vi "GDSProject_CreateClass.vi"(0 "Project Refnum In":refnum<vi>, 1 "Project Item To Create Class Below(Use MyComputer if not wired)":refnum<vi>, 2 "ClassFolder":path=path "C:/Documents and Settings/Micke/Mina dokument/LabView/8.1 Beta/Projects/ClassFiles/MyClass3.lvclass", 3 "ClassName":string, 5 "error in (no error)":errorcluster) -> (14 "Project Refnum Out":refnum<vi>, 15 "Class Refnum Out":refnum<vi>, 16 "ClassPathOut":path, 19 "error out":errorcluster)   [LabVIEW 2020]
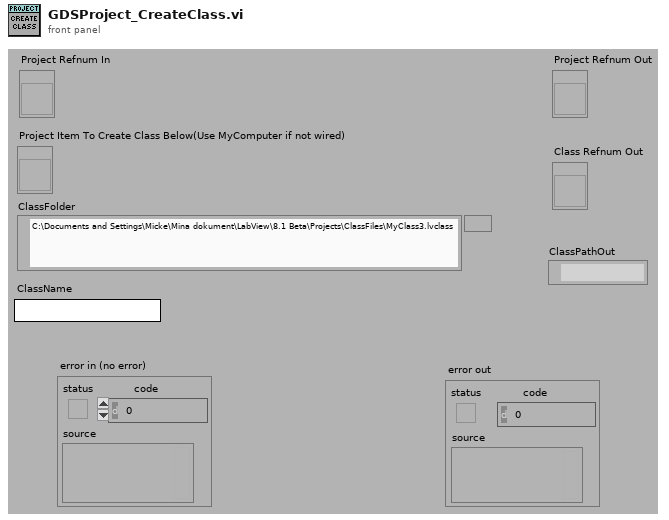
[diagram p1: front panel]
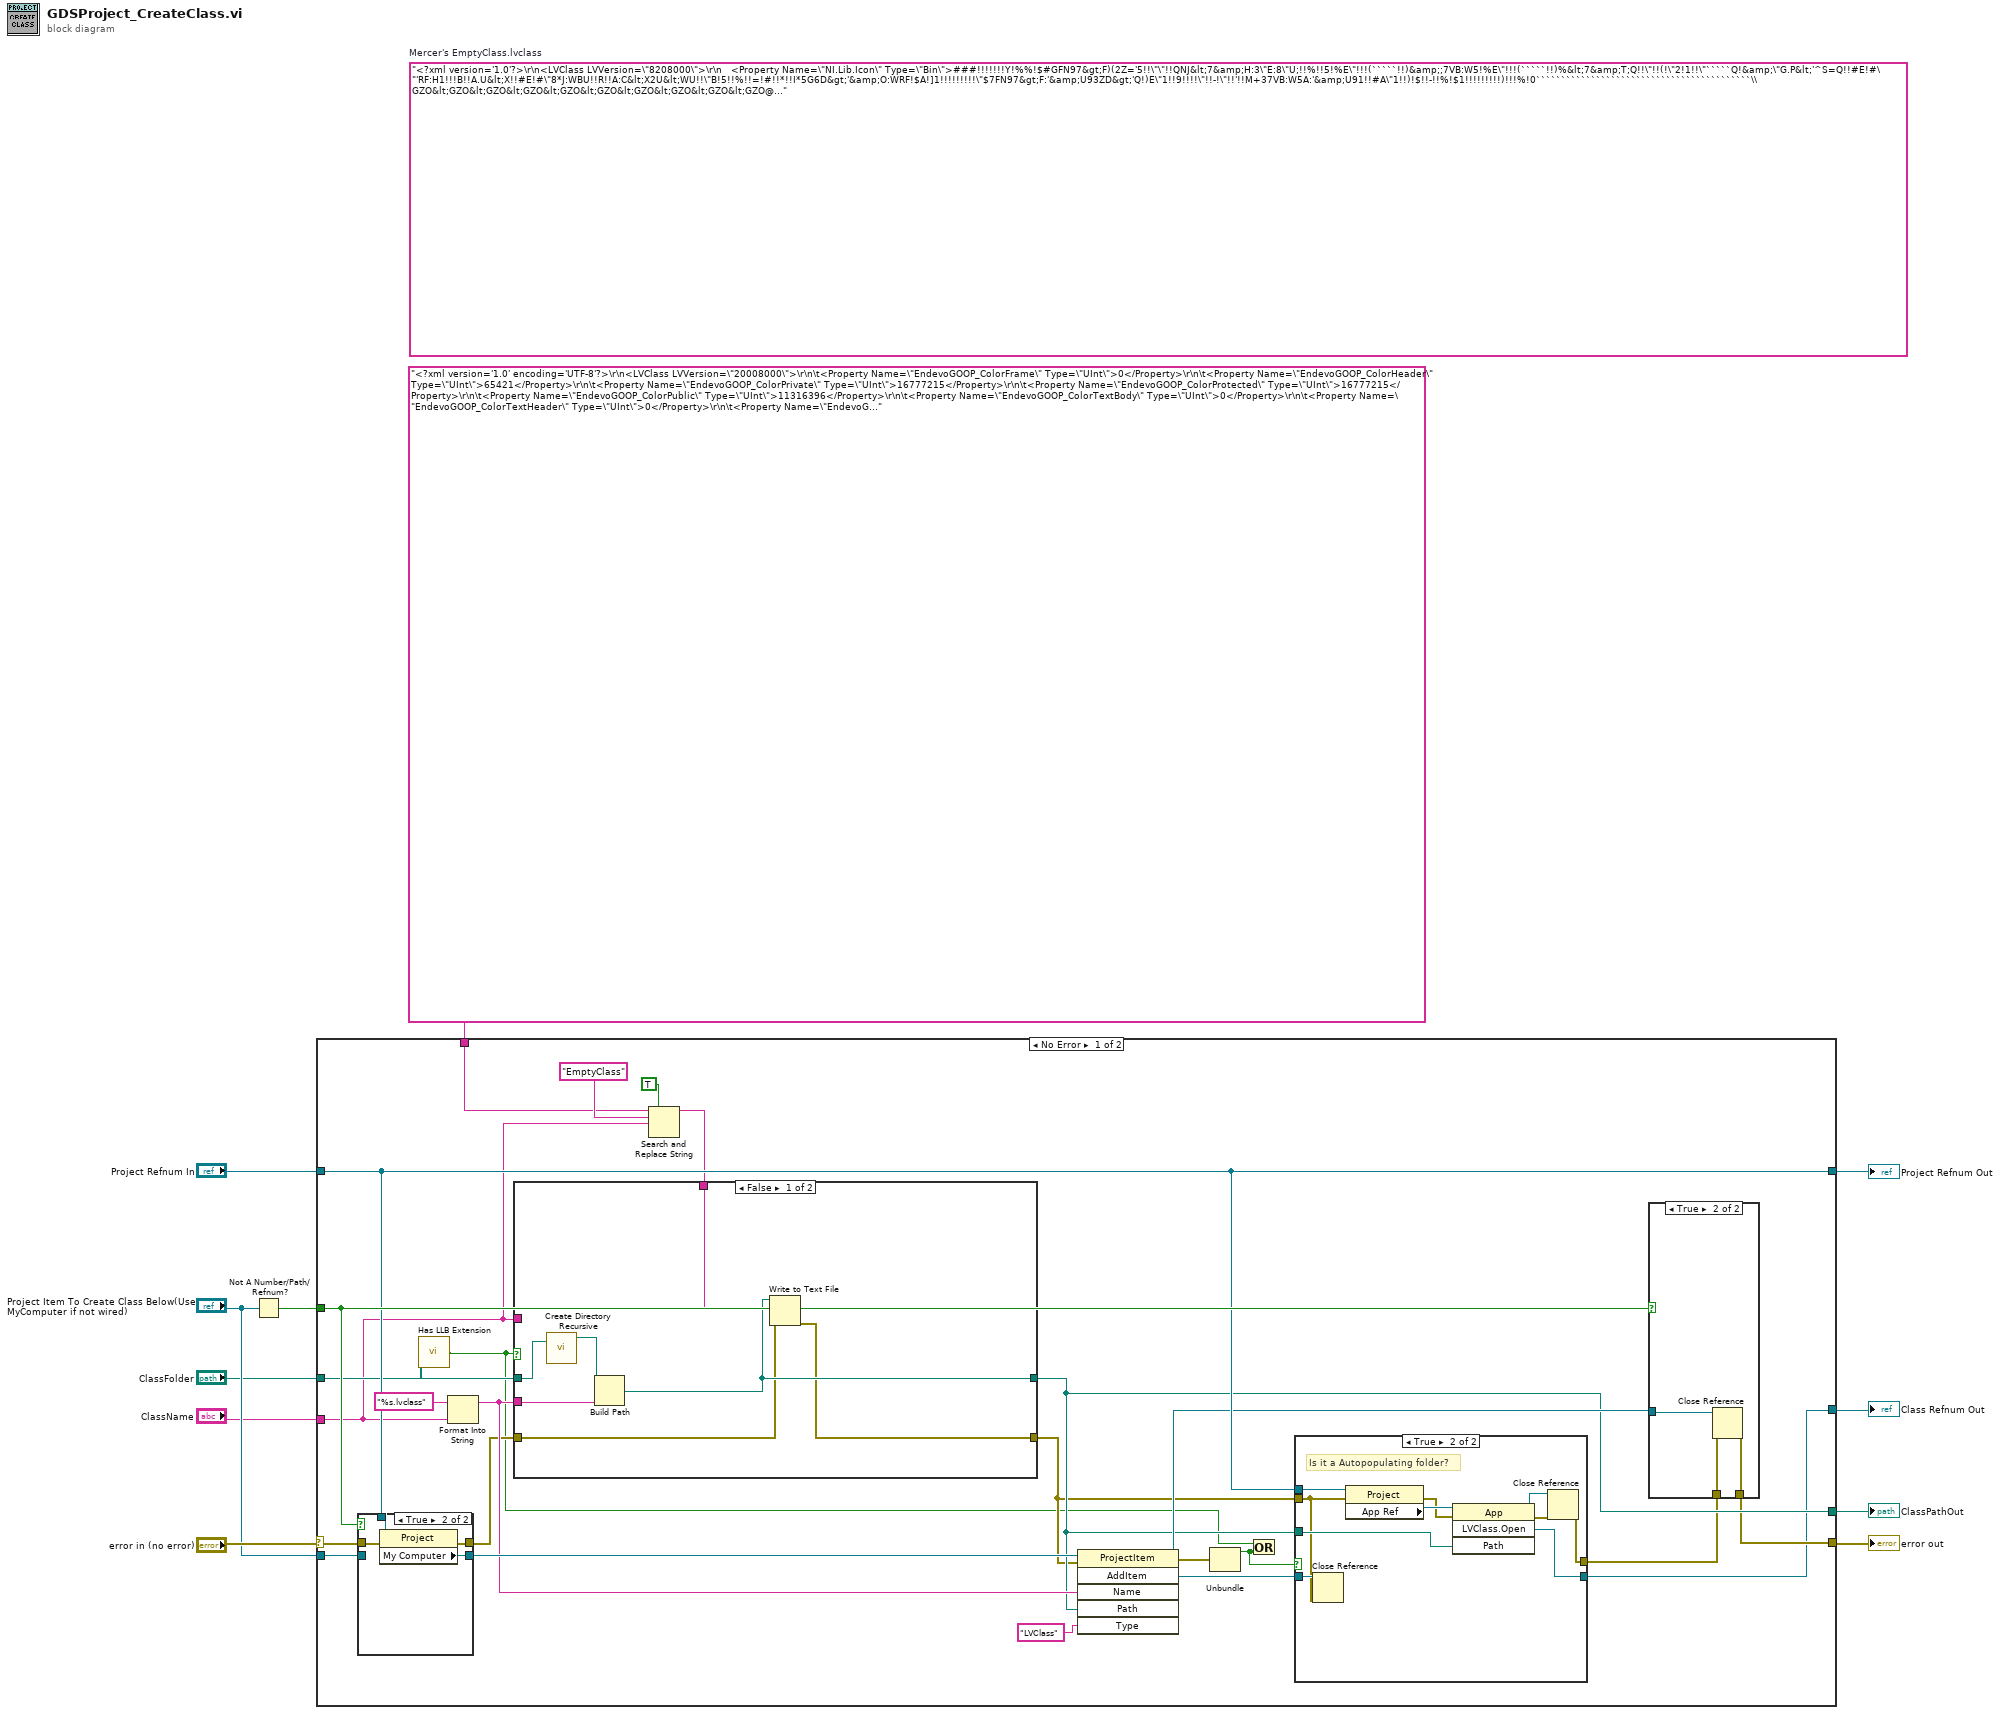
[diagram p0: block diagram]
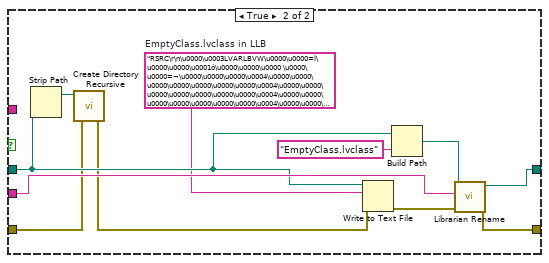
[diagram p2: hidden frame]
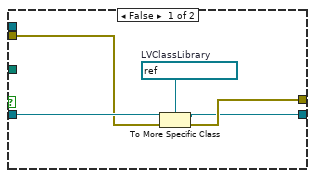
[diagram p3: hidden frame]
diagram:
  (unwired) "<?xml version='1.0'?>\r\n<LVClass LVVersion=\"8208000\">\r\n   <Property Name=\"NI.Lib.Icon\" Type=\"Bin\">###!!!!!!!Y!%%!$#GFN97&gt;F)(2Z='5!!\"\"!!QNJ&lt;7&amp;H:3\"E:8\"U;!!%!!5!%E\"!!!(`````!!)&amp;;7VB:W5!%E\"!!!(`````!!)%&lt;7&amp;T;Q!!\"!!(!\"2!1!!\"`````Q!&amp;\"G.P&lt;'^S=Q!!#E!#\"'RF:H1!!!B!!A.U&lt;X!!#E!#\"8*J:WBU!!R!!A:C&lt;X2U&lt;WU!!\"B!5!!%!!=!#!!*!!I*5G6D&gt;'&amp;O:WRF!$A!]1!!!!!!!!!\"$7FN97&gt;F:'&amp;U93ZD&gt;'Q!)E\"1!!9!!!!\"!!-!\"!!'!!M+37VB:W5A:'&amp;U91!!#A\"1!!)!$!!-!!%!$1!!!!!!!!!)!!!%!0```````````````````````````````````````````\\GZO&lt;GZO&lt;GZO&lt;GZO&lt;GZO&lt;GZO&lt;GZO&lt;GZO&lt;GZO&lt;GZO@``O&lt;GZO&lt;GZO&lt;GZO&lt;GZO&lt;GZO&lt;GZO&lt;GZO&lt;GZO&lt;GZ`\\GZ``_ZO&lt;GZO&lt;GZO&lt;GZO&lt;GZO&lt;GZO&lt;GZO&lt;GZO&lt;GZO@``O&lt;H``\\GZO&lt;GZO&lt;GZO&lt;GZO&lt;GZO&lt;GZO&lt;GZO&lt;GZO&lt;GZO@_ZO@``O&lt;GZO&lt;GZO&lt;GZO&lt;GZO&lt;GZO&lt;GZO&lt;GZO&lt;GZO&lt;GZ`\\GZ``_ZO&lt;GZO&lt;GZO&lt;GZO&lt;GZO&lt;GZO&lt;GZO&lt;GZO&lt;GZO&lt;H`O&lt;H``\\GZO&lt;GZO&lt;GZO&lt;GZO&lt;GZO&lt;GZO&lt;GZO&lt;GZO&lt;GZO@_ZO@``O&lt;GZO&lt;GZO&lt;GZO&lt;GZO&lt;GZO&lt;GZO&lt;GZO&lt;GZO&lt;GZ`\\GZ``_ZO&lt;GZO&lt;GZO&lt;GZO&lt;GZO&lt;GZO&lt;GZO&lt;GZO&lt;GZO@```\\H``\\GZO&lt;GZO&lt;GZO&lt;GZO&lt;GZO&lt;GZO&lt;GZO&lt;GZO&lt;GZO&lt;GZO@```\\H`O@_Z`\\H`O@_Z`\\H`O@_Z`\\H`O@_Z`\\H`O@_Z``]!!!!!!!!!!!!!!!!!!!!!!!!!!!!!!!!!!!!!!!$``Q$``````````````Q!!!!!!!!!!!!!!!!!!!!!!!0``!0^%2%2%`U2%2%4`!!!!!!!!!!!!!!!!!!!!!!!!``]!`U2%2%4`2%2%20]!!!!!!!!!!!!!!!!!!!!!!!$``Q$`2%2%20^%2%2%`Q!!!!!!!!!!!!!!!!!!!!!!!0``!0^%2%2%`U2%2%4`!!!!!!!!!!!!!!!!!!!!!!!!``]!``````````````]!!!!!!!!!!!!!!!!!!!!!!!$``Q$`!!!!!0]!!!!!AY-!!!!!!!!!!!!!!!!!!!!!!0``!0]!!!!!`Q!!!!#$\"9/$!!!!!!!!!!!!!!!!!!!!``]!`Q!!!!$`!#-D)Y-&amp;\"17$AQ!!!!!!!!!!!!!!!!$``Q$`!!!!!0]!!!!!AQ5&amp;`Q5&amp;AY-!!!!!!!!!!!!!!0``!0````````````_$\"@```Q5&amp;\"9-D)Q!!!!!!!!!!``]!!!!!!!!!!!!!!)-&amp;\"@]&amp;\"9/$!!!!!!!!!!!!!!$``Q!!!!!!!!!!V.45AQ5&amp;\"9/$!!!!!!!!!!!!!!!!!0``!!!!!!!!!!!!!!#$\"9/$!!!!!!!!!!!!!!!!!!!!``]!!!!!!!!!!!!!!)/$!!!!!!!!!!!!!!!!!!!!!!$``Q!!!!!!!!!!!!!!!!!!!!!!!!!!!!!!!!!!!!!!!0``!!!!!!!!!!!!!!!!!!!!!!!!!!!!!!!!!!!!!!!!``]!!!!!!!!!!!!!!!!!!!!!!!!!!!!!!!!!!!!!!!$```````````````````````````````````````````]!!!#!``````````````````````````````````````````````````````````````````````````````````````````````````````````````````````````````````````````````````````````````````````````]!!!%!!0```Q$``]Q!``_:!0``:A$``T-!``]!!0`-`Q$`T-Q!`]S:!0`-:A$`T$-!`]Q!!0_:`Q$`G=Q!`ZG:!0_::A$`G4-!`ZE!!0^G`Q$`:MQ!`W;:!0^G:A$`:D-!`W9!!0]T`Q$`-]Q!`T/:!0]T:A$`-T-!`T-!!0]!`Q$`!-Q!`Q#:!0]!:A$`!$-!`Q!!!-T``Q$-`]Q!T0_:!-T`:A$-`T-!T0]!!-T-`Q$-T-Q!T-S:!-T-:A$-T$-!T-Q!!-S:`Q$-G=Q!T*G:!-S::A$-G4-!T*E!!-RG`Q$-:MQ!T';:!-RG:A$-:D-!T'9!!-QT`Q$--]Q!T$/:!-QT:A$--T-!T$-!!-Q!`Q$-!-Q!T!#:!-Q!:A$-!$-!T!!!!*H``Q#:`]Q!G@_:!*H`:A#:`T-!G@]!!*H-`Q#:T-Q!G=S:!*H-:A#:T$-!G=Q!!*G:`Q#:G=Q!G:G:!*G::A#:G4-!G:E!!*FG`Q#::MQ!G7;:!*FG:A#::D-!G79!!*ET`Q#:-]Q!G4/:!*ET:A#:-T-!G4-!!*E!`Q#:!-Q!G1#:!*E!:A#:!$-!G1!!!'&lt;``Q\"G`]Q!:P_:!'&lt;`:A\"G`T-!:P]!!'&lt;-`Q\"GT-Q!:MS:!'&lt;-:A\"GT$-!:MQ!!';:`Q\"GG=Q!:JG:!';::A\"GG4-!:JE!!':G`Q\"G:MQ!:G;:!':G:A\"G:D-!:G9!!'9T`Q\"G-]Q!:D/:!'9T:A\"G-T-!:D-!!'9!`Q\"G!-Q!:A#:!'9!:A\"G!$-!:A!!!$0``Q!T`]Q!-`_:!$0`:A!T`T-!-`]!!$0-`Q!TT-Q!-]S:!$0-:A!TT$-!-]Q!!$/:`Q!TG=Q!-ZG:!$/::A!TG4-!-ZE!!$.G`Q!T:MQ!-W;:!$.G:A!T:D-!-W9!!$-T`Q!T-]Q!-T/:!$-T:A!T-T-!-T-!!$-!`Q!T!-Q!-Q#:!$-!:A!T!$-!-Q!!!!$``Q!!`]Q!!0_:!!$`:A!!`T-!!0]!!!$-`Q!!T-Q!!-S:!!$-:A!!T$-!!-Q!!!#:`Q!!G=Q!!*G:!!#::A!!G4-!!*E!!!\"G`Q!!:MQ!!';:!!\"G:A!!:D-!!'9!!!!T`Q!!-]Q!!$/:!!!T:A!!-T-!!$-!!!!!`Q!!!-Q!!!#:!!!!:A!!!$-!\\A!!!.U!!!#\\!!!!KA!!!)A!!!\"X!!!!61!!!%1!!!!C!!!!%1!!!!$O!!!!X1!!!,M!!!#K!!!!C!!!!(=!!!\"6!!!!2!!!!#)!!!!2!!!!!/Y!!!$&gt;!!!!OQ!!!+I!!!#)!!!!&gt;Q!!!&amp;5!!!\"%!!!!)A!!!\"%!\\O\\O!.X&gt;X1#\\O\\M!KKKK!)C)C!\"X&gt;X=!6666!%2%2!!C)C)!%2%2!!!!!!!!!!!!)!!A!!!!!!!!!!%!!!#!`````Y!!!!'!!!!*A!!!'9!!!!G!!!!*A!!!#9!!!!G!!!!*A!!!(9!!!!(`````A!!!!&lt;`Y!!'TG!!\"L7A!!;VI!!'TG!!\"P`!!!;%-!!'B?Q!\"I8D!!;%*)!'`[ZY\"A!EA!9\"YQ!'!?Q!\"A!Q!!9!!!!'!!!!\"A!!!!@````]!!!#!``````````````````````````````````````````````````````````````````````````````````````````````````````````````````````````````````````````````````````````````````````````]!!!!#!0```Q!!!!!!!!!!!#!!)!!!!!!</Property>\r\n   <Property Name=\"NI.Lib.Version\" Type=\"Str\">1.0.0.0</Property>\r\n   <Property Name=\"NI.LVClass.ClassNameVisibleInProbe\" Type=\"Bool\">true</Property>\r\n   <Property Name=\"NI.LVClass.FlattenedPrivateDataCTL\" Type=\"Bin\">###!!!!!!!)!\"!!&amp;!!Q!1!!\"`````Q!!!!%!!1!!%VB35V*$$1I!!UR71U.-1F:8!!!0_!!!!W!!!!!A!!!0W!!!!\"=!!!!\"%E6N=(2Z1WRB=X-O&lt;(:D&lt;'&amp;T=Q!!!!\"Q##'!!A!Q!!!)!!!!!!!!\"!!$!$Q!P!!@1!!#!!!!!!%!!1!'`````Q!!!!!!!!!!!!!!!!!!!!!!!!!!!!!!!!!!!!!!!!!'!!!!%!!!!!!!!!!!!!!!!!!!!!!!!!!!V\"W-W9]!MA4JA!G9\\0B#@A!!!']!!5R71U-B27VQ&gt;(F$&lt;'&amp;T=SZM&gt;G.M98.T/E6N=(2Z1WRB=X-O9X2M!!!!!!!\"!!*735R#!!!!!2*&amp;&lt;8\"U?5.M98.T,GRW9WRB=X-!5&amp;2)-!!!!\"E!!1!$!!!327VQ&gt;(F$&lt;'&amp;T=SZM&gt;G.M98.T!!-!!!!!7A!!!!%!5A$RQOG`-1!!!!)327VQ&gt;(F$&lt;'&amp;T=SZM&gt;G.M98.T$E6N=(2Z1WRB=X-O9X2M!$J!5!!!(5.M&gt;8.U:8)A&lt;W9A9WRB=X-A=(*J&gt;G&amp;U:3\"E982B!!%!!!!!!!!\";!!!!\"I!#A\"D!!!\"?!!%!!1!!Q!+!'1!!!!Q!!%!#!\"A!!!!$!!+!&amp;!!!A!#!!-!#A\"D!!!!-!!\"!!B!\"Q.G&lt;'=!#%!(!W^3&gt;!!)1!=$:7^G!\"\"!5!!$!!9!\"Q!)!X6E:A!E1&amp;!!!\"V$&lt;(6T&gt;'6S)'^G)'.M98.T)(\"S;8:B&gt;'5A:'&amp;U91!+1&amp;!!!!.E:G1!#E\"1!!!$&gt;(BE!!J!5!!!!W^M:!!+1&amp;!!!!.F?(1!%A\"1!!9!#1!+!!M!$!!.!!Y!#A\"D!!!!*!!\"!!9!AQ!+!!I!9Q!!!!A!\"!!+!'-!!!!!!!1!\"!!#!!1!!1!)!'!!!!!%!$Y!5!!=!\"1!&amp;!!6!\"5!&amp;1!6!!%!!1!\"!\"5!&amp;1!6!\"5!!1!\"!!%!!1!6!\"5!&amp;1!6!\"5!&amp;1!6!\"5!&amp;A!7!\"9!#A\"E!!!!!1!8!!1!!!!+!!!1!!!%%!%!\"2!!!!]1\"!!1%!!!%2!!!\")1!!!4%!!!'$!!!\"E1!!!!!%!!!!%)?*RD9-!*'\"E9G$9!;1[9Q(]AA)IX!'E7X&amp;L*\"V!\\-.DYR&amp;!\")V#?K14)9%;)A&gt;Q,&gt;D-=M+(J!A$&amp;D2/W!!!!-!!\"6EF%5S&amp;&amp;&lt;8\"U?5.M98.T,GRW9WRB=X-[27VQ&gt;(F$&lt;'&amp;T=SZD&gt;'Q!!!!!!!!!!Q!!!*Y!!!$E?*T,9W\"AS$3W-&amp;P&amp;A!$*_3GJ)0I#%(?_W'=)IAJYDDPI#!*:!;(&gt;LAT`\"8J46$BM19J+W8?!K--4`D_9-'&amp;#@&amp;R5:(4MY1GBX4EK(-'\"17(B/RC\"MJD#X;5-/]*\"\"LNJ\\&amp;!!UQY\\]M#U3Q:)2_A,E+EA7W\"[:Q(Z:Y&amp;3).H`1-$)Q-+AT&amp;$$U-,1A_2W:X]86S1OW!]!1%1X?!!!!!!!#QAAA!!!!!-Y,D)!!!!!!)$`````A!!!!9!!!!'!!!!\"A!Q!!9!T!!'!Q-!\"AQ!Q!91!#!''!!A\"B9!Y!92A[!'%'VA\"B!;I!91&amp;7!'%\"KA\"B!69!91'K!'%\"6]\"AQ;PQ9$&amp;8Q'!.PY\"A!`Y#9!\"Y\"G!!!!*A!!!#9!!!!G!!!!*A!!!#9!!!\"W!!!!\"`````Q!!\"!$```````````````````````````````````````````]!!!!!!!!!!!!!!!!!!!!!!!!!!!!!!!!!!!!!!!$``Q!!!!!!!!!!!!!!!!!!!!!!!!!!!!!!!!!!!!!!!0``!!!!!!!!!!!!!!!!!!!!!!!!!!!!!!!!!!!!!!!!``]!!!!!!!!!!!!!!*35!!!!!!!!!!!!!!!!!!!!!!$``Q!!!!!!!!!!!*3GI+;GF!!!!!!!!!!!!!!!!!!!!0``!!!!!!!!!*3GI*K;GJKGJJ1!!!!!!!!!!!!!!!!!``]!!!!!!*3GI*K;GJK;GJK;JK;5!!!!!!!!!!!!!!$``Q!!!!#GI*K;GJK;GJK;GJK;GK;G!!!!!!!!!!!!!0``!!!!!+#AGJK;GJK;GJK;GJK;L+9!!!!!!!!!!!!!``]!!!!!I+;GI*K;GJK;GJK;L+SMI!!!!!!!!!!!!!$``Q!!!!#AJK;GJK#;GJK;L+SML+SA!!!!!!!!!!!!!0``!!!!!+#GJK;GJK;AJKSML+SML+!!!!!!!!!!!!!!``]!!!!!I+;GJK;GJK;ML+SML+SMI!!!!!!!!!!!!!$``Q!!!!#AJK;GJK;GJKSML+SML+SA!!!!!!!!!!!!!0``!!!!!+#GJK;GJK;GL+SML+SML+!!!!!!!!!!!!!!``]!!!!!I+;GJK;GJK;ML+SML+SMI!!!!!!!!!!!!!$``Q!!!!#AJK;GJK;GJKSML+SML+SA!!!!!!!!!!!!!0``!!!!!+;GJK;GJK;GL+SML+SMJK9L+SM!!!!!!!!!``]!!!!!!+#AJK;GJK;ML+SMJK;A+SML+SML!!!!!!$``Q!!!!!!!!#AJK;GJKSMJK;A+SML+SML!!!!!!!!!0``!!!!!!!!!!!!I+;GJK;;+SML+SML+Q!!!!!!!!!!``]!!!!!!!!!!!!!!+#;+SML+SML+Q!!!!!!!!$`!!$``Q!!!!!!!!!!!!!!!!!!+SML+Q!!!!!!!!!!``]!!0``!!!!!!!!!!!!!!!!!!!!!!!!!!!!!!!!!!!!`Q!!``]!!!!!!!!!!!!!!!!!!!!!!!!!!!!!!!!!!!$`!!$``Q!!!!!!!!!!!!!!!!!!!!!!!!!!!!!!!!!!!0]!!0``!!!!!!!!!!!!!!!!!!!!!!!!!!!!!!!!!!!!`Q!!``]!!!!!!!!!!!!!!!!!!!!!!!!!!!!!!!!!!!$`!!$``Q!!!!!!!!!!!!!!!!!!!!!!!!!!!!!!!!!!````!0``!!!!!!!!!!!!!!!!!!!!!!!!!!!!!!!!!!!!!!!!````````````````````````````````````````````!!!!4!!!!!%!2!$RQOG`-1!!!!)(1WRB=X-A-1N$&lt;'&amp;T=S!R,G.U&lt;!!Q1&amp;!!!\"V$&lt;(6T&gt;'6S)'^G)'.M98.T)(\"S;8:B&gt;'5A:'&amp;U91!\"!!!!!!!Q!!!!!1!E1&amp;!!!\"V$&lt;(6T&gt;'6S)'^G)'.M98.T)(\"S;8:B&gt;'5A:'&amp;U91!$!!!!!!!!!!!!-!!\"2F\")5#&amp;&amp;&lt;8\"U?5.M98.T,GRW9WRB=X-[27VQ&gt;(F$&lt;'&amp;T=SZD&gt;'Q!!!!!!!!!!Q!!!&amp;!!!!!!!!!%\"!!!!!!!&amp;A!&amp;!#-!(A!!!\"9!!!!'!!!!)Q!!!\"Y!!!!!!1!!!!!!!!!!!!!!!!!!!!!!!!!!!!!!!!!!#A!!!!!!!!!%5'&amp;O:1!!!'E!!!!!!!!%\"!!!!!!!!Q!\"!\"!!C1!!!!-!!!!#!!!!%!!!!)E!!!!!!1!!!!!!!!!!!!!!!!!!!!!!!!!!!!!!!!!!#A!!!!!!!!!&gt;1WRV=X2F=C\"P:C\"D&lt;'&amp;T=S\"Q=GFW982F)'2B&gt;'%!!!!!!!\"1!!!!!!!!\"!1!!!!!!!%!!1!/!\"I!!!!\"!!!!!A!!!!Y!!!!;!!!!!!%!!!!!!!!!!!!!!!!!!!!!!!!!!!!!!!!!!!I!!!!!!!!!\"&amp;\"B&lt;G5!!!*X!!!&amp;&amp;HC=H:1`;\".2(-&gt;`\\Z,I3T$U*5WVQ5CCP,2&amp;UM7`.@CHVN?B5AI3#QY\"/RTI&amp;IJ5H&gt;LFFB1#!3'$U,&amp;:(4)I4E8C&gt;)O41TO%TCY/&amp;O8M8@S^/^`F'CY/8MDFXLXX_8X@\\`O_\"##7:J/;!ZMW%(;%$]MW*.AC0GT:-#%?J0=_*SH)KQ#&amp;9OYU`UC%G&gt;ZD3_1X!FHCE\"_:0,%\"?!(Y2?B?]B@4,&amp;WCCWR(=QD/H[5\\&lt;&amp;5SG3S/ZOEK/]#*H!VH^(W3@'3]\"Q,%_#,:\\F/P\"F[J&amp;5]GYE!;+1O!68\"L&amp;2MOO^6A5/?+W#&gt;%F?E@^Y_(SU\"]B2XC\\SGX8-+'[VD/K\"'=.W&lt;EH@=9@Z@D^6BXVC0(Y,ROHEM^:!XC;%^Y`C&gt;N&amp;'=VGH5,R'WY9;(7$(1[(&gt;[&lt;2F45Y:0(6P'T,MQ,GQI&amp;WBBQ.SX1&amp;$@F3MZ*L)LA/F2(9H-72)S;R\"2==O'%\"[/CK\\HFQ3,PP!H3NSS))NVKN23.['P6;F8KMB=+N?&gt;^^,E.:1NCP,?!;`P@U&amp;H]YNE?9L@@*4Y\"562?U]WJ6#;Y\\Y.C78-.DSL$&lt;Y=:(B&gt;V\"L+/*A]+NK8D#S==DQS;O#-&gt;LU'\\X=9G]#[&lt;E\"6/\\%39W;OB\"N[6PP]VU.0XU21/.U\"(&gt;.SX4Q^[=!`.&amp;\\]?0`.]5-'30KDB\"GQ&lt;JL&lt;'IL23H)ZQU3_7)])EO'9Y?'0`&amp;&lt;TII\"%W+HCE35JE6ZD*F[%'J%+$2UI)XC@.E6D[(]&amp;$P3&lt;#5P.6?0$'P?!&amp;[%$Q*-\\.%&lt;H,_,E,_KW/$.R&gt;\\W,O[,7BX%%!U@%)A\"ZVP`JPOMP_I`?(Q^`GD1`OU(&amp;&amp;*P]!ITNFNQ!!!!!)!!!!)!!!\"5A!!!!Q!!&amp;#2%B1)56N=(2Z1WRB=X-O&lt;(:D&lt;'&amp;T=TJ&amp;&lt;8\"U?5.M98.T,G.U&lt;!!!!!!!!!!$!!!!@!!!!*6YH'.A9*AI)-(UD[(O,Q/4Q&amp;=A1`IP!\\/A(_.P\"A:/0Y($1*J21*,Z(Y0M8Q&lt;W8QQ-ANJA'?UDOBQ-5+$+RKBCR?2SGIG\"1Z,DM#!(7!&amp;(CQ&lt;$````69I9Q2*@DVS$KT`C!W?W8!#2+L0E7X;!O@^!*)=%!&amp;UH)5E!!!!)!!!!\"Q!!!1!!!!$`!!!!\"!!!!\"J-6E.M98.T5(*J&gt;G&amp;U:52B&gt;'&amp;597*0=G2F=AABA!)!!!!#!!1!\"Q!-!%!!!@````]!!!!\"!!%!!!!!!!!!!!!!!\"N-6E.M98.T5(*J&gt;G&amp;U:52B&gt;'&amp;5;7VF=X2B&lt;8!))9!#!!!!!1!%!!=!!1!!QOG`-1!!!!!!!!!;4&amp;:$&lt;'&amp;T=V\"S;8:B&gt;'6%982B6(FQ:52F=W-))9!#!!!!!1!)!$$`````!!%!!!!!!!Y!!!!\"!!9!5!!!!!%!!!!!!!!!!!!?4&amp;:$&lt;'&amp;T=V\"S;8:B&gt;'6%982B2':M&gt;%2B&gt;'&amp;4;8JF##'!!A!!!!%!\"!!$!!%!!!!!!!!!!!!!!!!!!!1!!!\"!!!!!+!!!!!)!!!1!!!!!!1!!!!!!!!!!!!!!!!!!!!!!!!!!!!!!!!!!!!!!!!$`!!%!!A!$!!Y!!!$I!!Y%!!!!!!Y!ZQ$7!!!!\\Q!/\"!!!!!!/!/=!VA!!!09!$A1!!!!!$A$H!.9!!!!!!!!!!!!!!!!!!!!!!!!!!!!!!!!!!!!!!!!!!!!!!!!!!!!!!!!!!!!!!!!!!!!!!!!!!!!!!!!!!!!!!!!!!!!!!!!!!!!!!!!!!!!!!!!!!!!!!!!!!!!!!!!!!!!!!!!!!!!!!!!!!!!!!!!!!!!!!!!!!!!!!!!!!!!!!!!!!!!!!!!!!!!!!!!!!!!!!!!!!!!!!!!!!!!!!!!!`1!.B!#!!!!.!.!!O1:597BP&lt;7%'6'&amp;I&lt;WVB\"F2B;'^N91%R!&amp;*45E-.#A!$4&amp;:$1UR#6F=!!!`Y!!!$9!!!!#!!!!`9!!!!!!!!!!!!!!!A!!!!.!!!!!!!!!!84%F#4A!!!!!!!!%E4&amp;:45A!!!!!!!!%Y4%FW;1!!!!!!!!&amp;-1U^/5!!!!!!!!!&amp;A6%UY-!!!!!!!!!&amp;U2%:%5Q!!!!!!!!')4%FE=Q!!!!!!!!'=6EF$2!!!!!!!!!'Q&gt;G6S=Q!!!!!!!!(%35.04A!!!!!!!!(9;7.M/!!!!!!!!!(M1V\"$-A!!!!!!!!)!2&amp;2)5!!!!!!!!!)54%FG=!!!!!!!!!)I6&amp;*F9Q!!!!)!!!)]2F\")9A!!!!!!!!*Y2F\"421!!!!!!!!+-4%FC:!!!!!!!!!+A1E2)9A!!!!!!!!+U1E2421!!!!!!!!,)6EF55Q!!!!!!!!,=466*2!!!!!!!!!,Q3%F46!!!!!!!!!-%2F2\"1A!!!!!!!!-9!!!!!0````]!!!!!!!!!!$D'MAI!!!!!`````Q!!!!!!!!!=,-;S#A!!!!$`````!!!!!!!!!*!ARL)+!!!!!0````]!!!!!!!!\"\"\"4'MAI!!!!!`````Q!!!!!!!!&amp;E#-;S#A!!!!$`````!!!!!!!!!N$]R&lt;)+!!!!!0````]!!!!!!!!$&amp;0$&amp;MAI!!!!!`````Q!!!!!!!!.)Z-7S#A!!!!4`````!!!!!!!!!_T9R&lt;)+!!!!!0````]!!!!!!!!$`-T&amp;MAI!!!!!`````Q!!!!!!!!3!Q-7S#A!!!!$`````!!!!!!!!#)3UR&lt;)+!!!!!0````]!!!!!!!!)V+D&amp;MAI!!!!!`````Q!!!!!!!!E)H-7S#A!!!!,`````!!!!!!!!#4S1R&lt;)+!!!!!`````]!!!!!!!!*E)4&amp;MAI!!!!%`````Q!!!!!!!!I!?-7S#A!!!!$`````!!!!!!!!#F2MR&lt;)+!!!!!0````]!!!!!!!!-U'$&amp;MAI!!!!!`````Q!!!!!!!!T=6-7S#A!!!!$`````!!!!!!!!$2\")R&lt;)+!!!!!0````]!!!!!!!!.E$T&amp;MAI!!!!!`````Q!!!!!!!!W=--7S#A!!!!$`````!!!!!!!!$K!ER&lt;)+!!!!!0````]!!!!!!!!/K\"D&amp;MAI!!!#!`````Q!!!!!!!!\\5$-7S#A!!!!!</Property>\r\n   <Item Name=\"EmptyClass.ctl\" Type=\"Class Private Data\" URL=\"EmptyClass.lvclass/EmptyClass.ctl\">\r\n      <Property Name=\"NI.LibItem.Scope\" Type=\"Int\">2</Property>\r\n   </Item>\r\n</LVClass>\r\n"  # Mercer's EmptyClass.lvclass
  n1 = Not A Number/Path/Refnum?(number/path/refnum="Project Item To Create Class Below(Use MyComputer if not wired)") -> (NaN/Path/Refnum?=w8:bool)
  n2 = case shown="No Error" "error in (no error)" {
    selector: "error in (no error)" -> [w36 w81]
    tunnel: [w21 w81] -> w10
    tunnel: "Project Refnum In" -> [w30 w80]
    tunnel: w8 -> [w33 _]
    tunnel: "Project Item To Create Class Below(Use MyComputer if not wired)" -> [w35 _]
    tunnel: [w30 w80] -> w6
    tunnel: "ClassName" -> [w15 _]
    tunnel: "ClassFolder" -> [w20 _]
    tunnel: [w12 _] -> w2
    tunnel: [w26 _] -> w3
    tunnel: "﻿<?xml version='1.0' encoding='UTF-8'?>\r\n<LVClass LVVersion=\"20008000\">\r\n\t<Property Name=\"EndevoGOOP_ColorFrame\" Type=\"UInt\">0</Property>\r\n\t<Property Name=\"EndevoGOOP_ColorHeader\" Type=\"UInt\">65421</Property>\r\n\t<Property Name=\"EndevoGOOP_ColorPrivate\" Type=\"UInt\">16777215</Property>\r\n\t<Property Name=\"EndevoGOOP_ColorProtected\" Type=\"UInt\">16777215</Property>\r\n\t<Property Name=\"EndevoGOOP_ColorPublic\" Type=\"UInt\">11316396</Property>\r\n\t<Property Name=\"EndevoGOOP_ColorTextBody\" Type=\"UInt\">0</Property>\r\n\t<Property Name=\"EndevoGOOP_ColorTextHeader\" Type=\"UInt\">0</Property>\r\n\t<Property Name=\"EndevoGOOP_FrameThickness\" Type=\"UInt\">1</Property>\r\n\t<Property Name=\"NI.Lib.Icon\" Type=\"Bin\">)!#!!!!!!!)!\"1!&amp;!!!-!%!!!@````]!!!!\"!!%!!!,M!!!*Q(C=T:3`;BN\"%)@HYE\"3'),[1\")^A7(;1)I)]A2[B8G#A%J@%9T]\"JESL6!L12!#'[[=1C]AAF^!J%QA=0FON@JTMCUV#8B8=X@[`7:H0_WO4C3VFS,0J4\\6JE@&lt;WG_OWY&gt;J'F48?U,T;4V-[`XR7[8/1\\?&amp;(RI`&lt;6VW]^&gt;V4NS&lt;@HK;`V4\\&gt;&lt;1&gt;_J0*-8^3T;NK]JC0WS#V-H:_&gt;A]SNP\\/87==_P/7P\\DP6\\M+C]6C`I#@-R;,2XUSKM620^N0T[^;@F7.R_0W_M`H7Z_@/5[NP8`TN&lt;`H(OZ`SJC/&gt;`;^]T.PO@&gt;^WJ\\\\I.^K*Y]X\\Y(S^*`A`T;21JI8%2'%%U;I.&amp;9&gt;[)%?[)%?[)(O[)\\O[)\\O[)ZO[):O[):O[);O[)KO[)KO[)K?/LKA#\\KAMSL\"Z-&amp;%1&gt;'A1*!-CA38A#@A#8A#(LZ+Q\"0Q\"$Q\"4]\"$CA1]!5`!%`!%0!S4A#@A#8A#HI#(5IEE5E?(*_#BP$A]$I`$Y`!Y0%QJ$I]$Y%TG&amp;(;+A#'/[4QY0![0Q]/D/$Q/D]0D]$A]W/,Q/$Q/D]0D]$!EL9IHGK;DQU-:-8A-(I0(Y$&amp;Y+#U'D]&amp;D]\"A]\"A`4C=&amp;D]\"A1RI2'=2$%''1E'&amp;]-(I/(GRA]\"I`\"9`!90&amp;BJBSSN4%04&gt;(2Y&amp;\"[&amp;2_&amp;2?\"1?3ID#I`!I0!K0QE.:58A5(I6(Y6&amp;YG%I5(I6(Y6&amp;!F%G:8J2CSE!F32%5(D\\JN'D;*5]EGLJ)0LS3$[8EQS&lt;Z%%E_(*)X8@*G3NYES9MP?6%F,Z&lt;E2:$]YS2$3Y;20)HEQ5WCL,AOC2ER)I&lt;%A/A40;*,&gt;*KB`TBRN6L*=LG5W7QGI^&amp;)BM/B$!9$[@@\\UOPVJ.PN3K@4E5V\\3V_X9P.?+HG__PD[\\LLXL2B__HJ\\X@PS\\OLT^^N'X`AJTG[+]PSC+#`/C`,G&lt;\"U`8R8FHQ]&amp;B2[,O`+S`FW_Y@\\CRWV:8&amp;,L@&lt;'J`44?D@*-VP@N'PU&amp;0-%B!A!!!!!</Property>\r\n\t<Property Name=\"NI.Lib.SourceVersion\" Type=\"Int\">536903680</Property>\r\n\t<Property Name=\"NI.Lib.Version\" Type=\"Str\">1.0.0.0</Property>\r\n\t<Property Name=\"NI.LVClass.ClassNameVisibleInProbe\" Type=\"Bool\">true</Property>\r\n\t<Property Name=\"NI.LVClass.FlattenedPrivateDataCTL\" Type=\"Bin\">)!#!!!!!!!)!\"1!&amp;!!!-!%!!!@````]!!!!\"!!%!!\"5T5F.31QU+!!.-6E.$4%*76Q!!%*Q!!!38!!!!)!!!%(Q!!!!8!!!!!2*&amp;&lt;8\"U?5.M98.T,GRW9WRB=X-!!!!!I#!!A!!!-!!!#!!!!!!!!!1!!Q!]!,Q!(U#!!A!!!!!\"!!%!\"P````]!!!!!!!!!!!!!!!$/H;O(FY.&amp;4+)2CHA'B9U&gt;!!!!\"A!!!\"!!!!!!R5\"4GBK/YEGB[&gt;\\S\\&lt;]72.1&gt;D.G0!,)%[9!*G/TY1HY!!!!!!!!!!*'!X=K51B&gt;-B:-)ENPZ:*1\"!!!!`````^1&gt;D.G0!,)%[9!*G/TY1HY!!!!1\\+0=6]!H7HW2!0E;,ZZYL1!!!!1!!!!!!!!!*Q!\"4&amp;:$1Q!!!!%!!F:*4%)!!!!!5&amp;2)-!!!!!5!!1!\"!!!!!!)!!Q!!!!!#!!%!!!!!!#)!!!!=?*RD9'.A;G#YQ!$%D%$-V-$U!]D_!/)T!!\"I!1AW!!!!!!\"&amp;!!!\"'(C=9W$!\"0_\"!%AR-D!QH1$3,'DC9\"L'JC&lt;!:3YOO[$CT&amp;!XME*%'9&amp;C4(O!$#;1(+J?E(`!@E)\"&lt;&amp;D-\"A\"W^3A6!!!!!!!!$!!\"6EF%5Q!!!!!!!Q!!!5-!!!+=?*RT9'2AS$3W-'M!UMR!L-$1Q*#=HZ,+R1$E-U\"!#R-$R3!!;JY7GLDBA=.J1+$(,^]#ZH?\\K,!UV[DQ-*8S`3^2Y1BY!2*M0M*RO.MDZ\\CD$6A*2R:$&amp;E0!`]#-ZC-]9.X)_HV57!Q0.&amp;1K-Z1+(W]U9949%AAVBO8Q$J$)964\\A(IY$DZE[:U)&amp;OA%E:UBD\",(82BVR)$M8B\\'1)1\\U/Q,[Q;[-IMR$#&lt;@T8&lt;=110%0OYA!K%S)&amp;1&amp;B#I!54N!2.RB%,HW^&lt;V&gt;I(\"B1QI4\"SBO!'&amp;'\".:D9'1!/:]*#%'G`PH``\\].5)1*+K9)&amp;1/R6U,:'EB[4E,&amp;(*$M!?E&amp;G&gt;!,J$7A\\-F1&gt;A0583#RKU#[!-K_!YV0%0MR6\"W)`1J)#U$:(Y(U!3D\\'Z4&gt;!)U.&gt;.L:X]56/5X!UBM!`Z2KE!!!!!!/)!'!\"Q!!\"D)Q,D!O-1!!!!!!!!QA!)!!!!!%-D!O-!!!!!!/)!'!\"Q!!\"D)Q,D!O-1!!!!!!!!QA!)!!!!!%-D!O-!!!!!!/)!'!\"Q!!\"D)Q,D!O-1!!!!!!!\"1\"!!!!^6=VAHEGIIQO=V*/\"EEZH1!!!!U!!!!!!!!!!!!!!!!!!!!!!!!!A0````_!!!!\"BE-=Y9F%I1')2ZD\"C53%)9:UO='!!!!\"`````Y!!!!'!!!!\"A!0!!9!--!'!-!Q\"A-!$!9$!!Q'!]!]\"A0Q`!9$``Q'!``]\"A0``!9$``Q'!``]\"A0``!9$``_'!@``ZA\"``Y9!(X]'!!8]\"A!!]!9!!!!(`````!!!#!0`````````````````````YC)C)C)C)C)C)C)C)C)C0_)C0_)_)C0_)D`_)``C)D`C)_)_0C)_)_0C)DYC)C)`YC0C)DYC0``C0_)D`C)C0_)DYDY_)DYDYC)_)C0C)D`C)D`C0`Y_)_0`YD`_)C)`YC)C)C)C)C)C)C)C)C)C0``````````````````````T-T-T-T-T-T-T-T-T-T-`]T-T-T-T-RXT-T-T-T-T0`-T-T-T-RZ[:@-T-T-T-T`T-T-T-RZ[)C*F]T-T-T-`]T-T-RZ[)C)C)G8T-T-T0`-T-T*[)C)C)C)C:T-T-T`T-T-TOC)C)C)C)_=T-T-`]T-T-[:[)C)C)``\\-T-T0`-T-T/G:HIC)```_T-T-T`T-T-TJG:G?H````MT-T-`]T-T-[:G:G@````\\-T-T0`-T-T/G:G:H````_T-T-T`T-T-TJG:G:`````MT-T-`]T-T-[:G:G@````\\-T-T0`-T-T/G:G:H````_T-T-T`T-T-S:G:G:````G@`]T-`]T-T-TOG:G@``G?````T0`-T-T-T/G:H`G?````T-T`T-T-T-T-[:G9`````-T-`]T-T-T-T-TI`````-T-T0`-T-T-T-T-T-```-T-T-T`T-T-T-T-T-T-T-T-T-T-``````````````````````!!!%!0```````````````````````````````````````````\\;WNL;WNL;WNL;WNL;WNL;WNL;WNL;WNL;WNL;WNP``NL;WNP``NL&lt;`NL;WNP``NL;W````NL&lt;```_WNL;W``_WNL&lt;`NL&lt;`NP_WNL&lt;`NL&lt;`NP_WNL;W`\\;WNL;WNL&lt;``\\;WNP_WNL;W`\\;WNP````_WNP``NL;W``_WNL;WNP``NL;W`\\;W`\\&lt;`NL;W`\\;W`\\;WNL&lt;`NL;WNP_WNL;W``_WNL;W``_WNP```\\&lt;`NL&lt;`NP```\\;W````NL;WNL&lt;``\\;WNL;WNL;WNL;WNL;WNL;WNL;WNL;WNL;WNL;WNP`````````````````````````````````````````````Y_0DY_0DY_0DY_0DY_0DY_0DY_0DY_0DY_0DY_0D```DY_0DY_0DY_0DY_0DYN&lt;8Y_0DY_0DY_0DY_0DY_0``_0DY_0DY_0DY_0DYN=3^R-3V_0DY_0DY_0DY_0DY```Y_0DY_0DY_0DYN=3^NL;WNM4%N@DY_0DY_0DY_0D```DY_0DY_0DYN=3^NL;WNL;WNL&lt;%R,8Y_0DY_0DY_0``_0DY_0DY_-3^NL;WNL;WNL;WNL;WR-4Y_0DY_0DY```Y_0DY_0DYP&lt;WWNL;WNL;WNL;WNL&lt;1R0DY_0DY_0D```DY_0DY_0C^R-3^NL;WNL;WNL&lt;1U.#^_0DY_0DY_0``_0DY_0DY_,X%R-4%P&lt;;WNL&lt;1U.$1U,XY_0DY_0DY```Y_0DY_0DYP=4%R-4%R,X%U.$1U.$1P@DY_0DY_0D```DY_0DY_0C^R-4%R-4%R.$1U.$1U.#^_0DY_0DY_0``_0DY_0DY_,X%R-4%R-4%U.$1U.$1U,XY_0DY_0DY```Y_0DY_0DYP=4%R-4%R-41U.$1U.$1P@DY_0DY_0D```DY_0DY_0C^R-4%R-4%R.$1U.$1U.#^_0DY_0DY_0``_0DY_0DY_,X%R-4%R-4%U.$1U.$1U,XY_0DY_0DY```Y_0DY_0DYR-4%R-4%R-41U.$1U.$%R+SML0DY_0D```DY_0DY_0DYP&lt;X%R-4%R.$1U.$%R,WML+SML+TY_0``_0DY_0DY_0DY_,X%R-4%U.$%R,WML+SML+TY_0DY```Y_0DY_0DY_0DY_0C^R-4%R,;ML+SML+SM_0DY_0D```DY_0DY_0DY_0DY_0DYP&lt;;ML+SML+SM_0DY_0DY_0``_0DY_0DY_0DY_0DY_0DY_0CML+SM_0DY_0DY_0DY```Y_0DY_0DY_0DY_0DY_0DY_0DY_0DY_0DY_0DY_0D```````````````````````````````````````````]!!!!#!!%!!!!!!!Q!!5:13&amp;!!!!!!!!-!!!!%!!!!!!!!!H=!!!4I?*SNF-VL%V%5R?]&lt;2HE*FLSEV89A*&lt;']RC)*C+,79,496[&amp;3CB),,IIG/0%$7C0Z%%&amp;I.Y/123%A:#&amp;WY3:&lt;&amp;VFU+R,=T+9L&amp;_UC&amp;0Q$X\"2&amp;/UHPGW1S-&gt;7Y-10$-.T@08@O/8E![F=WJD2BT1,#^P&amp;BQ1+P&lt;B+!?IR#ZR&gt;Z$7S*`!)SIB%,:OA3WV7;*'D\"#&gt;W-U(/C\".][V32\"XL-^,$X/.'TGN=#HG[0_7\\T\"_)=A,RVTOPIAS$:)5\\H(1^`JBJ&amp;&amp;14#GZ.U@)UUAYL3K'B/XU]]S\"J&gt;P04'KW3U^&amp;D\"B$O6YYQRW2/F0&gt;EN3*F'5\\L1%&lt;$E&amp;N6L.B@RN+'+0-9U-C&gt;LDFA=Q!7'/ZXED;D.?GU'&gt;B+-D1MUX=H9*^;0$QG3))P@375X5U2)B;_;0X\"-,2HDD\"N8IHLZ$BOY97U#!V\"`1VF&lt;LH?4^C^)&amp;OT;!2ET'#5PC=^+#MY;JJ*AKN215+U,:NE&amp;V&lt;,AK&lt;&lt;BJW_!2*1;O$_6`_#$5_M4Y\\%IR8]DEQNF(Y9=L[8Q_`$TX^%7[E!HL[5,[K%-*97I8Z.&gt;,M89YBE'&amp;,+2[NZW&amp;;L7+#]#\\CVZ$&gt;*1XOJQ07_&gt;\"\\WZ=&gt;T=H6&gt;X.8=@.C2^X(]PN4=96*\\0AJP5]JN80_A@[,;U8`X^;,W')VPL3#MNYL1Z)XO5WZ+96[Q&amp;798E!-YX-?G^;WSK/TK#U8DG36MHWJ&lt;63K@3H.&gt;Z*K^ABJ\"V79\\NVU$L!S')-6&lt;A0+4OSY&amp;HM':TO@CZWTR;;Z+*&amp;N&lt;]8M$H57L@AJ*A.@'4T]A^!Z_E=WU24]41[24@J@PV,^`3J,X2*9ZO]5H\\SNS%[&gt;AC[@FY8!!!!!!1!!!!A!!!!\"!!!!!!!!!!-!!&amp;#2%B1!!!!!!!$!!!!\"!!!!!!!!!\"F!!!!&gt;8C=9W\"A+\"3190L(50?8A5HA+Z!B`:?\"7&gt;#0]4=$![?@Q'%AT3AA#237`=P!,KA.&amp;N9_IMP\"!!7K&lt;)Q=EBS(\"4H!-BQN'AT```^8+7,E_(LE'FT2%2]Y5W770)=%!'5)':I!!!!!!!!%!!!!\"Q!!!=1!!!!'!!!!)6^O;6^-98.U3WZP&gt;WZ0&gt;WZJ&lt;G&gt;-6E.M98.T1WRV=X2F=A!!!$9A!)!!!!!!!1!)!$$`````!!%!!!!!!\"I!!!!\"!\"*!5!!!#E6N=(2Z1WRB=X-!!!%!!!!!!!!!!!!;4&amp;:$&lt;'&amp;T=V\"S;8:B&gt;'6%982B6'&amp;C4X*E:8)!!!!F)!#!!!!!!!)!\"1!(!!!-!%!!!@````]!!!!\"!!%!!!!!!!!!!!!!!\"N-6E.M98.T5(*J&gt;G&amp;U:52B&gt;'&amp;5;7VF=X2B&lt;8!!!!!:)!#!!!!!!!%!\"1!(!!!\"!!$DN\\2R!!!!!!!!!#:-6E.M98.T5(*J&gt;G&amp;U:52B&gt;'&amp;-98.U18\"Q&lt;'FF:&amp;2J&lt;76T&gt;'&amp;N=!!!!\"EA!)!!!!!!!1!&amp;!!=!!!%!!//XN(%!!!!!!!!!'ER71WRB=X.1=GFW982F2'&amp;U962Z='6%:8.D!!!!.C!!A!!!!!!\"!!A!-0````]!!1!!!!!!'A!!!!%!%E\"1!!!+27VQ&gt;(F$&lt;'&amp;T=Q!!!1!!!!!!!!!!!\"Z-6E.M98.T5(*J&gt;G&amp;U:52B&gt;'&amp;%:GRU2'&amp;U96.J?G5!!!!:)!#!!!!!!!%!\"1!$!!!\"!!!!!!!!!!!!!!!!!!1!!A!)!!!!\"!!!!%!!!!!I!!!!!A!!\"!!!!!!#!!!!!!!!!!!!!!!!!!!!!!!!!!!!!!!!!!!!!!!!!.U!!!&amp;6?*S.E%&amp;/!E%126^0K]!AC,AW[95,6GSYQ#1%VY14/'&amp;GD%G&lt;1;9BM/.1*B\\)#_A.`$.A.(&amp;D@F*&gt;^&lt;PK`_I'&lt;FDQ_@\\W_A*%Q^HT+OSH0KWKM&gt;]O[\\0`CVI'TSC:Q_X5&lt;[K1LVV:O+&lt;,L&gt;:0WT4E,EN$SLF!4!&lt;G![0#HEIG3DN*#VPY2^L*Q:;,=#4SMG!A&lt;;PW#VJWER8%N:=.OUT4=S,;&gt;,D\\FX^%)[.AU.C$L-_YFYDDEJ\\)'HW:@=/=]*@ZO&lt;FK=(S)93\"&amp;N*#_46F-FWO'CNUPE7%W91!!!!!!!'5!!1!#!!-!\"!!!!%A!$Q1!!!!!$Q$:!.1!!!\"2!!]%!!!!!!]!W1$5!!!!7A!0\"!!!!!!0!.E!V!!!!'-!$91!A!!!$1$5!-1)5W6H&lt;W5A65E)5W6H&lt;W5A65E)5W6H&lt;W5A65E\"-1!!!&amp;*45E-.#A!$4&amp;:$1UR#6F=!!\"#=!!!%FQ!!!#!!!\"\"]!!!!!!!!!!!!!!!A!!!!.!!!\")A!!!!@4%F#4A!!!!!!!!'%4&amp;:45A!!!!!!!!'95F242Q!!!!!!!!'M1U.46!!!!!!!!!(!4%FW;1!!!!!!!!(51U^/5!!!!!!!!!(I6%UY-!!!!!!!!!(]2%:%5Q!!!!!!!!)14%FE=Q!!!!!!!!)E6EF$2!!!!!!!!!)Y&gt;G6S=Q!!!!1!!!*-5U.45A!!!!!!!!+Q2U.15A!!!!!!!!,%35.04A!!!!!!!!,9;7.M.!!!!!!!!!,M;7.M/!!!!!!!!!-!1V\"$-A!!!!!!!!-54%FG=!!!!!!!!!-I2F\"&amp;?!!!!!!!!!-]2F\")9A!!!!!!!!.12F\"421!!!!!!!!.E6F\"%5!!!!!!!!!.Y4%FC:!!!!!!!!!/-1E2&amp;?!!!!!!!!!/A1E2)9A!!!!!!!!/U1E2421!!!!!!!!0)6EF55Q!!!!!!!!0=2&amp;2)5!!!!!!!!!0Q466*2!!!!!!!!!1%3%F46!!!!!!!!!196E.55!!!!!!!!!1M2F2\"1A!!!!!!!!2!!!!!!0````]!!!!!!!!!!!!!!!!!!!!!!!!!!!!!!!!!!!!=!!!!!!!!!!$`````!!!!!!!!!-!!!!!!!!!!!0````]!!!!!!!!!V!!!!!!!!!!!`````Q!!!!!!!!$=!!!!!!!!!!$`````!!!!!!!!!1A!!!!!!!!!!0````]!!!!!!!!\"%!!!!!!!!!!!`````Q!!!!!!!!%Y!!!!!!!!!!$`````!!!!!!!!!91!!!!!!!!!!0````]!!!!!!!!\"F!!!!!!!!!!%`````Q!!!!!!!!,=!!!!!!!!!!@`````!!!!!!!!!P!!!!!!!!!!#0````]!!!!!!!!$!!!!!!!!!!!*`````Q!!!!!!!!-5!!!!!!!!!!L`````!!!!!!!!!S1!!!!!!!!!!0````]!!!!!!!!$/!!!!!!!!!!!`````Q!!!!!!!!.1!!!!!!!!!!$`````!!!!!!!!!W1!!!!!!!!!!0````]!!!!!!!!$[!!!!!!!!!!!`````Q!!!!!!!!8M!!!!!!!!!!$`````!!!!!!!!#@!!!!!!!!!!!0````]!!!!!!!!*_!!!!!!!!!!!`````Q!!!!!!!!I)!!!!!!!!!!$`````!!!!!!!!#B!!!!!!!!!!!0````]!!!!!!!!-D!!!!!!!!!!!`````Q!!!!!!!!S5!!!!!!!!!!$`````!!!!!!!!$*Q!!!!!!!!!!0````]!!!!!!!!-L!!!!!!!!!!!`````Q!!!!!!!!SU!!!!!!!!!!$`````!!!!!!!!$3!!!!!!!!!!!0````]!!!!!!!!.+!!!!!!!!!!!`````Q!!!!!!!!\\Q!!!!!!!!!!$`````!!!!!!!!$PA!!!!!!!!!!0````]!!!!!!!!0!!!!!!!!!!!!`````Q!!!!!!!!]M!!!!!!!!!)$`````!!!!!!!!%\"!!!!!!$E6N=(2Z1WRB=X-O9X2M!!!!!!</Property>\r\n\t<Property Name=\"NI.LVClass.Geneology\" Type=\"Xml\"><String>\r\r\n<Name></Name>\r\r\n<Val>!!!!!2*&amp;&lt;8\"U?5.M98.T,GRW9WRB=X-!5&amp;2)-!!!!!!!!!!!!!!!!1!\"!!!!!!!!!!!!!!%!%E\"1!!!+27VQ&gt;(F$&lt;'&amp;T=Q!!!1!!!!!!!!!!!!!\"$ERB9F:*26=A4W*K:7.U!&amp;\"53$!!!!!!!!!!!!!A!)!!!!!!!!!!!!!!!!</Val>\r\r\n</String>\r\r\n</Property>\r\n\t<Property Name=\"NI.LVClass.IsTransferClass\" Type=\"Bool\">false</Property>\r\n\t<Property Name=\"NI.LVClass.LowestCompatibleVersion\" Type=\"Str\">1.0.0.0</Property>\r\n\t<Property Name=\"NI.SortType\" Type=\"Int\">3</Property>\r\n\t<Property Name=\"NI_IconEditor\" Type=\"Str\">50 48 48 49 56 48 48 55 13 0 0 0 0 1 23 21 76 111 97 100 32 38 32 85 110 108 111 97 100 46 108 118 99 108 97 115 115 0 0 1 0 0 0 0 0 9 0 0 25 66 1 100 1 100 80 84 72 48 0 0 0 4 0 0 0 0 0 0 12 30 0 29 0 0 12 24 0 0 12 0 0 0 0 0 0 32 0 32 0 24 0 0 0 0 0 255 255 255 0 0 255 255 255 255 255 255 255 255 255 255 255 255 255 255 255 255 255 255 255 255 255 255 255 255 255 255 255 255 255 255 255 255 255 255 255 255 255 255 255 255 255 255 255 255 255 255 255 255 255 255 255 255 255 255 255 255 255 255 255 255 255 255 255 255 255 255 255 255 255 255 255 255 255 255 255 255 255 255 255 255 255 255 255 255 255 255 255 255 255 255 255 255 255 255 255 255 255 255 255 255 255 255 255 255 255 255 255 255 255 255 255 255 255 255 255 255 255 255 255 255 255 255 255 255 255 255 255 255 255 255 255 255 255 255 255 255 255 255 255 255 255 255 255 255 255 255 255 255 255 255 255 255 255 255 255 255 255 255 255 255 255 255 255 255 255 255 255 255 255 255 255 255 255 255 255 255 255 255 255 255 255 255 255 255 255 255 255 255 255 255 255 255 255 255 255 255 255 255 255 255 255 255 255 255 255 255 255 255 255 255 255 255 255 255 255 255 255 255 255 255 255 255 255 255 255 255 255 255 255 255 255 255 255 255 255 255 255 255 255 255 255 255 255 255 255 255 255 255 255 255 255 255 255 255 255 255 255 255 255 255 255 255 255 255 255 255 255 255 255 255 255 255 255 255 255 255 255 255 255 255 255 255 255 255 255 255 255 255 255 255 255 255 255 255 255 255 255 255 255 255 255 255 255 255 255 255 255 255 255 255 255 255 255 255 255 255 255 255 255 255 255 255 255 255 255 255 255 255 255 255 255 255 255 255 255 255 255 255 255 255 255 255 255 255 255 255 255 255 255 255 255 255 255 255 255 255 255 255 255 255 255 255 255 255 255 255 255 255 255 255 255 255 255 255 255 255 255 255 255 255 255 255 255 255 255 255 255 255 255 255 255 255 255 255 255 255 255 255 255 255 255 255 255 255 255 255 255 255 255 255 255 255 255 255 255 255 255 255 255 255 255 255 255 255 255 255 255 255 255 255 255 255 255 255 255 255 255 255 255 255 255 255 255 255 255 255 255 255 255 255 255 255 255 255 255 255 255 255 255 255 255 255 255 255 255 255 255 255 255 255 255 255 255 255 255 255 255 255 255 255 255 255 255 255 255 255 255 255 255 255 255 255 255 255 255 255 255 255 255 255 255 255 255 255 255 255 255 255 255 255 255 255 255 255 255 255 255 255 255 255 255 255 255 255 255 255 255 255 255 255 255 255 255 255 255 255 255 255 255 255 255 255 255 255 255 255 255 255 255 255 255 255 255 255 255 255 255 255 255 255 255 255 255 255 255 255 255 255 255 255 255 255 255 255 255 255 255 255 255 255 255 255 255 255 255 255 255 255 255 255 255 255 255 255 255 255 255 255 255 255 255 255 255 255 255 255 255 255 255 255 255 255 255 255 255 255 255 255 255 255 255 255 255 255 255 255 255 255 255 255 255 255 255 255 255 255 255 255 255 255 255 255 255 255 255 255 255 255 255 255 255 255 255 255 255 255 255 255 255 255 255 255 255 255 255 255 255 255 255 255 255 255 255 255 255 255 255 255 255 255 255 255 255 255 255 255 255 255 255 255 255 255 255 255 255 255 255 255 255 255 255 255 255 255 255 255 255 255 255 255 255 255 255 255 255 255 255 255 255 255 255 255 255 255 255 255 255 255 255 255 255 255 255 255 255 255 255 255 255 255 255 255 255 255 255 255 255 255 255 255 255 255 255 255 255 255 255 255 255 255 255 255 255 255 255 255 255 255 255 255 255 255 255 255 255 255 255 255 255 255 255 255 255 255 255 255 255 255 255 255 255 255 255 255 255 255 255 255 255 255 255 255 255 255 255 255 255 255 255 255 255 255 255 255 255 255 255 255 255 255 255 255 255 255 255 255 255 255 255 255 255 255 255 255 255 255 255 255 255 255 255 255 255 255 255 255 255 255 255 255 255 255 255 255 255 255 255 255 255 255 255 255 255 255 255 255 255 255 255 255 255 255 255 255 255 255 255 255 255 255 255 255 255 255 255 255 255 255 255 255 255 255 255 255 255 255 255 255 255 255 255 255 255 255 255 255 255 255 255 255 255 255 255 255 255 255 255 255 255 255 255 255 255 255 255 255 255 255 255 255 255 255 255 255 255 255 255 255 255 255 255 255 255 255 255 255 255 255 255 255 255 255 255 255 255 255 255 255 255 255 255 255 255 255 255 255 255 255 255 255 255 255 255 255 255 255 255 255 255 255 255 255 255 255 255 255 255 255 255 255 255 255 255 255 255 255 255 255 255 255 255 255 255 255 255 255 255 255 255 255 255 255 255 255 255 255 255 255 255 255 255 255 255 255 255 255 255 255 255 255 255 255 255 255 255 255 255 255 255 255 255 255 255 255 255 255 255 255 255 255 255 255 255 255 255 255 255 255 255 255 255 255 255 255 255 255 255 255 255 255 255 255 255 255 255 255 255 255 255 255 255 255 255 255 255 255 255 255 255 255 255 255 255 255 255 255 255 255 255 255 255 255 255 255 255 255 255 255 255 255 255 255 255 255 255 255 255 255 255 255 255 255 255 255 255 255 255 255 255 255 255 255 255 255 255 255 255 255 255 255 255 255 255 255 255 255 255 255 255 255 255 255 255 255 255 255 255 255 255 255 255 255 255 255 255 255 255 255 255 255 255 255 255 255 255 255 255 255 255 255 255 255 255 255 255 255 255 255 255 255 255 255 255 255 255 255 255 255 255 255 255 255 255 255 255 255 255 255 255 255 255 255 255 255 255 255 255 255 255 255 255 255 255 255 255 255 255 255 255 255 255 255 255 255 255 255 255 255 255 255 255 255 255 255 255 255 255 255 255 255 255 255 255 255 255 255 255 255 255 255 255 255 255 255 255 255 255 255 255 255 255 255 255 255 255 255 255 255 255 255 255 255 255 255 255 255 255 255 255 255 255 255 255 255 255 255 255 255 255 255 255 255 255 255 255 255 255 255 255 255 255 255 255 255 255 255 255 255 255 255 255 255 255 255 255 255 255 255 255 255 255 255 255 255 255 255 255 255 255 255 255 255 255 255 255 255 255 255 255 255 255 255 255 255 255 255 255 255 255 255 255 255 255 255 255 255 255 255 255 255 255 255 255 255 255 255 255 255 255 255 255 255 255 255 255 255 255 255 255 255 255 255 255 255 255 255 255 255 255 255 255 255 255 255 255 255 255 255 255 255 255 255 255 255 255 255 255 255 255 255 255 255 255 255 255 255 255 255 255 255 255 255 255 255 255 255 255 255 255 255 255 255 255 255 255 255 255 255 255 255 255 255 255 255 255 255 255 255 255 255 255 255 255 255 255 255 255 255 255 255 255 255 255 255 255 255 255 255 255 255 255 255 255 255 255 255 255 255 255 255 255 255 255 255 255 255 255 255 255 255 255 255 255 255 255 255 255 255 255 255 255 255 255 255 255 255 255 255 255 255 255 255 255 255 255 255 255 255 255 255 255 255 255 255 255 255 255 255 255 255 255 255 255 255 255 255 255 255 255 255 255 255 255 255 255 255 255 255 255 255 255 255 255 255 255 255 255 255 255 255 255 255 255 255 255 255 255 255 255 255 255 255 255 255 255 255 255 255 255 255 255 255 255 255 255 255 255 255 255 255 255 255 255 255 255 255 255 255 255 255 255 255 255 255 255 255 255 255 255 255 255 255 255 255 255 255 255 255 255 255 255 255 255 255 255 255 255 255 255 255 255 255 255 255 255 255 255 255 255 255 255 255 255 255 255 255 255 255 255 255 255 255 255 255 255 255 255 255 255 255 255 255 255 255 255 255 255 255 255 255 255 255 255 255 255 255 255 255 255 255 255 255 255 255 255 255 255 255 255 255 255 255 255 255 255 255 255 255 255 255 255 255 255 255 255 255 255 255 255 255 255 255 255 255 255 255 255 255 255 255 255 255 255 255 255 255 255 255 255 255 255 255 255 255 255 255 255 255 255 255 255 255 255 255 255 255 255 255 255 255 255 255 255 255 255 255 255 255 255 255 255 255 255 255 255 255 255 255 255 255 255 255 255 255 255 255 255 255 255 255 255 255 255 255 255 255 255 255 255 255 255 255 255 255 255 255 255 255 255 255 255 255 255 255 255 255 255 255 255 255 255 255 255 255 255 255 255 255 255 255 255 255 255 255 255 255 255 255 255 255 255 255 255 255 255 255 255 255 255 255 255 255 255 255 255 255 255 255 255 255 255 255 255 255 255 255 255 255 255 255 255 255 255 255 255 255 255 255 255 255 255 255 255 255 255 255 255 255 255 255 255 255 255 255 255 255 255 255 255 255 255 255 255 255 255 255 255 255 255 255 255 255 255 255 255 255 255 255 255 255 255 255 255 255 255 255 255 255 255 255 255 255 255 255 255 255 255 255 255 255 255 255 255 255 255 255 255 255 255 255 255 255 255 255 255 255 255 255 255 255 255 255 255 255 255 255 255 255 255 255 255 255 255 255 255 255 255 255 255 255 255 255 255 255 255 255 255 255 255 255 255 255 255 255 255 255 255 255 255 255 255 255 255 255 255 255 255 255 255 255 255 255 255 255 255 255 255 255 255 255 255 255 255 255 255 255 255 255 255 255 255 255 255 255 255 255 255 255 255 255 255 255 255 255 255 255 255 255 255 255 255 255 255 255 255 255 255 255 255 255 255 255 255 255 255 255 255 255 255 255 255 255 255 255 255 255 255 255 255 255 255 255 255 255 255 255 255 255 255 255 255 255 255 255 255 255 255 255 255 255 255 255 255 255 255 255 255 255 255 255 255 255 255 255 255 255 255 255 255 255 255 255 255 255 255 255 255 255 255 255 255 255 255 255 255 255 255 255 255 255 255 255 255 255 255 255 255 255 255 255 255 255 255 255 255 255 255 255 255 255 255 255 255 255 255 255 255 255 255 255 255 255 255 255 255 255 255 255 255 255 255 255 255 255 255 255 255 255 255 255 255 255 255 255 255 255 255 255 255 255 255 255 255 255 255 255 255 255 255 255 255 255 255 255 255 255 255 255 255 255 255 255 255 255 255 255 255 255 255 255 255 255 255 255 255 255 255 255 255 255 255 255 255 255 255 255 255 255 255 255 255 255 255 255 255 255 255 255 255 255 255 255 255 255 255 255 255 255 255 255 255 255 255 255 255 255 255 255 255 255 255 255 255 255 255 255 255 255 255 255 255 255 255 255 255 255 255 255 255 255 255 255 255 255 255 255 255 255 255 255 255 255 255 255 255 255 255 255 255 255 255 255 255 255 255 255 255 255 255 255 255 255 255 255 255 255 255 255 255 255 255 255 255 255 255 255 255 255 255 255 255 255 255 255 255 255 255 255 255 255 255 255 255 255 255 255 255 255 255 255 255 255 255 255 255 255 255 255 255 255 255 255 255 255 255 255 255 255 255 255 255 255 255 255 255 255 255 255 255 255 255 255 255 255 255 255 255 255 255 255 255 255 255 255 255 255 255 255 255 255 255 255 255 255 255 255 255 255 255 255 255 255 255 255 255 255 255 255 255 255 255 255 255 255 255 255 255 255 255 255 255 255 255 255 255 255 255 255 255 255 255 255 255 255 255 255 255 255 255 255 255 255 255 255 255 255 255 255 255 255 255 255 255 255 255 255 255 255 255 255 255 255 255 255 255 255 255 255 255 255 255 255 255 255 255 255 255 255 255 255 255 255 255 255 255 255 255 255 255 255 255 255 255 255 255 255 255 255 255 255 255 255 255 255 255 255 255 255 255 255 255 255 255 255 255 255 255 255 255 255 255 255 255 255 255 255 255 255 255 255 255 255 255 255 255 255 255 255 255 255 255 255 255 255 255 255 255 255 255 255 255 255 255 255 255 255 255 255 255 255 255 255 255 255 255 255 255 255 255 255 255 255 255 255 255 255 255 255 255 255 255 255 255 255 255 255 255 255 255 255 255 255 255 255 255 255 255 255 255 255 255 255 255 255 255 255 255 255 255 255 255 255 255 255 255 255 255 255 255 255 255 255 255 255 255 255 255 255 255 255 255 255 255 255 255 255 255 255 255 255 255 255 255 255 255 255 255 255 255 255 255 255 255 255 255 255 255 255 255 255 255 255 255 255 255 255 255 255 255 255 255 255 255 255 255 255 255 255 255 255 255 255 255 255 255 255 255 255 255 255 255 255 255 255 255 255 255 255 255 255 255 255 255 255 255 255 255 255 255 255 255 255 255 255 255 255 255 255 255 255 255 255 255 255 255 255 255 255 255 255 255 255 255 255 255 255 255 255 255 255 255 255 255 255 255 255 255 255 255 255 255 255 255 255 255 255 255 255 255 255 255 255 255 255 255 255 255 255 255 255 255 255 255 255 255 255 255 255 255 255 255 255 255 255 255 255 255 255 255 255 255 255 255 255 255 255 255 255 255 255 255 255 255 255 255 255 255 255 255 255 255 255 255 255 255 255 255 255 255 255 255 255 255 255 255 255 255 255 255 255 255 255 255 255 255 255 255 255 255 255 255 255 255 255 255 255 255 255 255 255 255 255 255 255 255 255 255 255 255 255 255 255 255 255 255 255 255 255 255 255 255 255 255 255 255 255 255 255 255 255 255 255 255 255 255 255 255 255 255 255 255 255 255 255 255 255 255 255 255 255 255 255 255 255 255 255 255 255 255 255 255 255 255 255 255 255 255 255 255 255 255 255 255 255 255 255 255 255 255 255 255 255 255 255 255 255 255 255 255 255 255 255 255 255 255 255 255 255 255 255 255 255 255 255 255 255 255 255 255 255 255 255 255 255 255 255 255 255 255 255 255 255 255 255 255 255 255 255 255 255 255 255 255 255 255 255 255 255 255 255 255 255 255 255 255 255 255 255 255 255 255 255 255 255 255 255 255 255 255 255 255 255 255 255 255 255 255 255 255 255 255 255 255 255 255 255 255 255 255 255 255 255 255 255 255 255 255 255 255 255 255 255 0 0 0 1 0 0 0 1 15 13 76 97 121 101 114 46 108 118 99 108 97 115 115 0 0 1 0 0 0 0 0 7 0 0 12 184 0 0 0 0 0 0 0 0 0 0 12 158 0 40 0 0 12 152 0 0 12 0 0 0 0 0 0 32 0 32 0 24 0 0 0 0 0 255 255 255 0 0 0 0 0 0 0 0 0 0 0 0 0 0 0 0 0 0 0 0 0 0 0 0 0 0 0 0 0 0 0 0 0 0 0 0 0 0 0 0 0 0 0 0 0 0 0 0 0 0 0 0 0 0 0 0 0 0 0 0 0 0 0 0 0 0 0 0 0 0 0 0 0 0 0 0 0 0 0 0 0 0 0 0 0 0 0 0 0 0 0 0 0 0 0 0 0 0 0 0 0 0 255 153 0 255 153 0 255 153 0 255 153 0 255 153 0 255 153 0 255 153 0 255 153 0 255 153 0 255 153 0 255 153 0 255 153 0 255 153 0 255 153 0 255 153 0 255 153 0 255 153 0 255 153 0 255 153 0 255 153 0 255 153 0 255 153 0 255 153 0 255 153 0 255 153 0 255 153 0 255 153 0 255 153 0 255 153 0 255 153 0 0 0 0 0 0 0 255 153 0 255 153 0 255 153 0 255 153 0 0 0 0 0 0 0 255 153 0 255 153 0 0 0 0 255 153 0 255 153 0 255 153 0 255 153 0 0 0 0 0 0 0 255 153 0 255 153 0 255 153 0 0 0 0 0 0 0 0 0 0 255 153 0 255 153 0 0 0 0 0 0 0 0 0 0 255 153 0 255 153 0 255 153 0 255 153 0 0 0 0 0 0 0 255 153 0 255 153 0 255 153 0 0 0 0 255 153 0 255 153 0 0 0 0 255 153 0 0 0 0 255 153 0 255 153 0 255 153 0 0 0 0 255 153 0 255 153 0 0 0 0 255 153 0 0 0 0 255 153 0 255 153 0 255 153 0 255 153 0 0 0 0 255 153 0 255 153 0 255 153 0 255 153 0 255 153 0 255 153 0 255 153 0 0 0 0 0 0 0 255 153 0 255 153 0 255 153 0 0 0 0 255 153 0 255 153 0 255 153 0 255 153 0 0 0 0 255 153 0 255 153 0 255 153 0 0 0 0 0 0 0 0 0 0 0 0 0 255 153 0 255 153 0 0 0 0 0 0 0 255 153 0 255 153 0 255 153 0 0 0 0 0 0 0 255 153 0 255 153 0 255 153 0 255 153 0 255 153 0 0 0 0 0 0 0 255 153 0 255 153 0 255 153 0 0 0 0 255 153 0 255 153 0 0 0 0 255 153 0 0 0 0 255 153 0 255 153 0 255 153 0 0 0 0 255 153 0 255 153 0 0 0 0 255 153 0 255 153 0 255 153 0 255 153 0 0 0 0 255 153 0 255 153 0 255 153 0 255 153 0 0 0 0 255 153 0 255 153 0 255 153 0 255 153 0 0 0 0 0 0 0 255 153 0 255 153 0 255 153 0 255 153 0 0 0 0 0 0 0 255 153 0 255 153 0 0 0 0 0 0 0 0 0 0 255 153 0 0 0 0 255 153 0 255 153 0 0 0 0 255 153 0 0 0 0 0 0 0 0 0 0 255 153 0 255 153 0 0 0 0 0 0 0 0 0 0 255 153 0 255 153 0 255 153 0 255 153 0 255 153 0 0 0 0 0 0 0 255 153 0 255 153 0 255 153 0 255 153 0 255 153 0 255 153 0 255 153 0 255 153 0 255 153 0 255 153 0 255 153 0 255 153 0 255 153 0 255 153 0 255 153 0 255 153 0 255 153 0 255 153 0 255 153 0 255 153 0 255 153 0 255 153 0 255 153 0 255 153 0 255 153 0 255 153 0 255 153 0 255 153 0 255 153 0 255 153 0 0 0 0 0 0 0 0 0 0 0 0 0 0 0 0 0 0 0 0 0 0 0 0 0 0 0 0 0 0 0 0 0 0 0 0 0 0 0 0 0 0 0 0 0 0 0 0 0 0 0 0 0 0 0 0 0 0 0 0 0 0 0 0 0 0 0 0 0 0 0 0 0 0 0 0 0 0 0 0 0 0 0 0 0 0 0 0 0 0 0 0 0 0 0 0 0 0 0 255 255 255 255 255 255 255 255 255 255 255 255 255 255 255 255 255 255 255 255 255 255 255 255 255 255 255 255 255 255 255 255 255 255 255 255 255 255 255 255 255 255 255 255 255 255 255 255 255 255 255 255 255 255 255 255 255 255 255 255 255 255 255 255 255 255 255 255 255 255 255 255 255 255 255 255 255 255 255 255 255 255 255 255 255 255 255 255 255 255 255 255 255 255 255 255 255 255 255 255 255 255 255 255 255 255 255 255 255 255 255 255 255 255 255 255 255 255 255 255 255 255 255 255 255 255 255 255 255 255 255 255 255 255 255 255 255 255 255 255 255 255 255 255 255 255 255 255 255 255 255 255 255 255 255 255 255 255 255 255 255 255 255 255 255 255 255 255 255 255 255 255 255 255 255 255 255 255 255 255 255 255 255 255 255 255 255 255 255 255 255 255 255 255 255 255 255 255 255 255 255 255 255 255 255 255 255 255 255 255 255 255 255 255 255 255 255 255 255 255 255 255 255 255 255 255 255 255 255 255 255 255 255 255 255 255 255 255 255 255 255 255 255 255 255 255 255 255 255 255 255 255 255 255 255 255 255 255 255 255 255 255 255 255 255 255 255 255 255 255 255 255 255 255 255 255 255 255 255 255 255 255 255 255 255 255 255 255 255 255 255 255 255 255 255 255 255 255 255 255 255 255 255 255 255 255 255 255 255 255 255 255 255 255 255 255 255 255 255 255 255 255 255 255 255 255 255 255 255 255 255 255 255 255 255 255 255 255 255 255 255 255 255 255 255 255 255 255 255 255 255 255 255 255 255 255 255 255 255 255 255 255 255 255 255 255 255 255 255 255 255 255 255 255 255 255 255 255 255 255 255 255 255 255 255 255 255 255 255 255 255 255 255 255 255 255 255 255 255 255 255 255 255 255 255 255 255 255 255 255 255 255 255 255 255 255 255 255 255 255 255 255 255 255 255 255 255 255 255 255 255 255 255 255 255 255 255 255 255 255 255 255 255 255 255 255 255 255 255 255 255 255 255 255 255 255 255 255 255 255 255 255 255 255 255 255 255 255 255 255 255 255 255 255 255 255 255 255 255 255 255 255 255 255 255 255 255 255 255 255 255 255 255 255 255 255 255 255 255 255 255 255 255 255 255 255 255 255 255 255 255 255 255 255 255 255 255 255 255 255 255 255 255 255 255 255 255 255 255 255 255 255 255 255 255 255 255 255 255 255 255 255 255 255 255 255 255 255 255 255 255 255 255 255 255 255 255 255 255 255 255 255 255 255 255 255 255 255 255 255 255 255 255 255 255 255 255 255 255 255 255 255 255 255 255 255 255 255 255 255 255 255 255 255 255 255 255 255 255 255 255 255 255 255 255 255 255 255 255 255 255 255 255 255 255 255 255 255 255 255 255 255 255 255 255 255 255 255 255 255 255 255 255 255 255 255 255 255 255 255 255 255 255 255 255 255 255 255 255 255 255 255 255 255 255 255 255 255 255 255 255 255 255 255 255 255 255 255 255 255 255 255 255 255 255 255 255 255 255 255 255 255 255 255 255 255 255 255 255 255 255 255 255 255 255 255 255 255 255 255 255 255 255 255 255 255 255 255 255 255 255 255 255 255 255 255 255 255 255 255 255 255 255 255 255 255 255 255 255 255 255 255 255 255 255 255 255 255 255 255 255 255 255 255 255 255 255 255 255 255 255 255 255 255 255 255 255 255 255 255 255 255 255 255 255 255 255 255 255 255 255 255 255 255 255 255 255 255 255 255 255 255 255 255 255 255 255 255 255 255 255 255 255 255 255 255 255 255 255 255 255 255 255 255 255 255 255 255 255 255 255 255 255 255 255 255 255 255 255 255 255 255 255 255 255 255 255 255 255 255 255 255 255 255 255 255 255 255 255 255 255 255 255 255 255 255 255 255 255 255 255 255 255 255 255 255 255 255 255 255 255 255 255 255 255 255 255 255 255 255 255 255 255 255 255 255 255 255 255 255 255 255 255 255 255 255 255 255 255 255 255 255 255 255 255 255 255 255 255 255 255 255 255 255 255 255 255 255 255 255 255 255 255 255 255 255 255 255 255 255 255 255 255 255 255 255 255 255 255 255 255 255 255 255 255 255 255 255 255 255 255 255 255 255 255 255 255 255 255 255 255 255 255 255 255 255 255 255 255 255 255 255 255 255 255 255 255 255 255 255 255 255 255 255 255 255 255 255 255 255 255 255 255 255 255 255 255 255 255 255 255 255 255 255 255 255 255 255 255 255 255 255 255 255 255 255 255 255 255 255 255 255 255 255 255 255 255 255 255 255 255 255 255 255 255 255 255 255 255 255 255 255 255 255 255 255 255 255 255 255 255 255 255 255 255 255 255 255 255 255 255 255 255 255 255 255 255 255 255 255 255 255 255 255 255 255 255 255 255 255 255 255 255 255 255 255 255 255 255 255 255 255 255 255 255 255 255 255 255 255 255 255 255 255 255 255 255 255 255 255 255 255 255 255 255 255 255 255 255 255 255 255 255 255 255 255 255 255 255 255 255 255 255 255 255 255 255 255 255 255 255 255 255 255 255 255 255 255 255 255 255 255 255 255 255 255 255 255 255 255 255 255 255 255 255 255 255 255 255 255 255 255 255 255 255 255 255 255 255 255 255 255 255 255 255 255 255 255 255 255 255 255 255 255 255 255 255 255 255 255 255 255 255 255 255 255 255 255 255 255 255 255 255 255 255 255 255 255 255 255 255 255 255 255 255 255 255 255 255 255 255 255 255 255 255 255 255 255 255 255 255 255 255 255 255 255 255 255 255 255 255 255 255 255 255 255 255 255 255 255 255 255 255 255 255 255 255 255 255 255 255 255 255 255 255 255 255 255 255 255 255 255 255 255 255 255 255 255 255 255 255 255 255 255 255 255 255 255 255 255 255 255 255 255 255 255 255 255 255 255 255 255 255 255 255 255 255 255 255 255 255 255 255 255 255 255 255 255 255 255 255 255 255 255 255 255 255 255 255 255 255 255 255 255 255 255 255 255 255 255 255 255 255 255 255 255 255 255 255 255 255 255 255 255 255 255 255 255 255 255 255 255 255 255 255 255 255 255 255 255 255 255 255 255 255 255 255 255 255 255 255 255 255 255 255 255 255 255 255 255 255 255 255 255 255 255 255 255 255 255 255 255 255 255 255 255 255 255 255 255 255 255 255 255 255 255 255 255 255 255 255 255 255 255 255 255 255 255 255 255 255 255 255 255 255 255 255 255 255 255 255 255 255 255 255 255 255 255 255 255 255 255 255 255 255 255 255 255 255 255 255 255 255 255 255 255 255 255 255 255 255 255 255 255 255 255 255 255 255 255 255 255 255 255 255 255 255 255 255 255 255 255 255 255 255 255 255 255 255 255 255 255 255 255 255 255 255 255 255 255 255 255 255 255 255 255 255 255 255 255 255 255 255 255 255 255 255 255 255 255 255 255 255 255 255 255 255 255 255 255 255 255 255 255 255 255 255 255 255 255 255 255 255 255 255 255 255 255 255 255 255 255 255 255 255 255 255 255 255 255 255 255 255 255 255 255 255 255 255 255 255 255 255 255 255 255 255 255 255 255 255 255 255 255 255 255 255 255 255 255 255 255 255 255 255 255 255 255 255 255 255 255 255 255 255 255 255 255 255 255 255 255 255 255 255 255 255 255 255 255 255 255 255 255 255 255 255 255 255 255 255 255 255 255 255 255 255 255 255 255 255 255 255 255 255 255 255 255 255 255 255 255 255 255 255 255 255 255 255 255 255 255 255 255 255 255 255 255 255 255 255 255 255 255 255 255 255 255 255 255 255 255 255 255 255 255 255 255 255 255 255 255 255 255 255 255 255 255 255 255 255 255 255 255 255 255 255 255 255 255 255 255 255 255 255 255 255 255 255 255 255 255 255 255 255 255 255 255 255 255 255 255 255 255 255 255 255 255 255 255 255 255 255 255 255 255 255 255 255 255 255 255 255 255 255 255 255 255 255 255 255 255 255 255 255 255 255 255 255 255 255 255 255 255 255 255 255 255 255 255 255 255 255 255 255 255 255 255 255 255 255 255 255 255 255 255 255 255 255 255 255 255 255 255 255 255 255 255 255 255 255 255 255 255 255 255 255 255 255 255 255 255 255 255 255 255 255 255 255 255 255 255 255 255 255 255 255 255 255 255 255 255 255 255 255 255 255 255 255 255 255 255 255 255 255 255 255 255 255 255 255 255 255 255 255 255 255 255 255 255 255 255 255 255 255 255 255 255 255 255 255 255 255 255 255 255 255 255 255 255 255 255 255 255 255 255 255 255 255 255 255 255 255 255 255 255 255 255 255 255 255 255 255 255 255 255 255 255 255 255 255 255 255 255 255 255 255 255 255 255 255 255 255 255 255 255 255 255 255 255 255 255 255 255 255 255 255 255 255 255 255 255 255 255 255 255 255 255 255 255 255 255 255 255 255 255 255 255 255 255 255 255 255 255 255 255 255 255 255 255 255 255 255 255 255 255 255 255 255 255 255 255 255 255 255 255 255 255 255 255 255 255 255 255 255 255 255 255 255 255 255 255 255 255 255 255 255 255 255 255 255 255 255 255 255 255 255 255 255 255 255 255 255 255 255 255 255 255 255 255 255 255 255 255 255 255 255 255 255 255 255 255 255 255 255 255 255 255 255 255 255 255 255 255 255 255 255 255 255 255 255 255 255 255 255 255 255 255 255 255 255 255 255 255 255 255 255 255 255 255 255 255 255 255 255 255 255 255 255 255 255 255 255 255 255 255 255 255 255 255 255 255 255 255 255 255 255 255 255 255 255 255 255 255 255 255 255 255 255 255 255 255 255 255 255 255 255 255 255 255 255 255 255 255 255 255 255 255 255 255 255 255 255 255 255 255 255 255 255 255 255 255 255 255 255 255 255 255 255 255 255 255 255 255 255 255 255 255 255 255 255 255 255 255 255 255 255 255 255 255 255 255 255 255 255 255 255 255 255 255 255 255 255 255 255 255 255 255 255 255 255 255 255 255 255 255 255 255 255 255 255 255 255 255 255 255 255 255 255 255 255 255 255 255 0 0 0 0 0 0 0 0 0 0 0 0 0 0 0 0 0 0 0 0 0 0 0 0 0 0 0 0 0 0 0 0 0 0 0 0 0 0 0 0 0 0 0 0 0 0 0 0 0 0 0 0 0 0 0 0 0 0 0 0 0 0 0 0 0 0 0 0 0 0 0 0 0 0 0 0 0 0 0 0 0 0 0 0 0 0 0 0 0 0 0 0 0 0 0 6 72 69 65 68 69 82 100 1 0 0 0 0 0 0 0 0 0 0 0 0 0 0 0 0 0 0 0 0 0 0 0 0 0 0 0 0 0 0 0 0 0 0 0 0 0 11 83 109 97 108 108 32 70 111 110 116 115 0 1 8 1 1\r\r\n</Property>\r\n\t<Item Name=\"EmptyClass.ctl\" Type=\"Class Private Data\" URL=\"EmptyClass.ctl\">\r\n\t\t<Property Name=\"NI.LibItem.Scope\" Type=\"Int\">2</Property>\r\n\t</Item>\r\n</LVClass>\r\n" ("text") -> [w13 _]
    frame No Error {
      n3 = case shown="True" w33 {
        tunnel: w30 -> [_ w79]
        tunnel: w36 -> [w74 w78]
        tunnel: [w75 w77] -> w32
        tunnel: w35 -> [w75 _]
        tunnel: [w74 w76] -> w24
        frame False {
        }
        frame True {
          n4 = property class="Project"(reference=w79, error in=w78) -> (error out=w76:errorcluster, "My Computer"=w77:refnum<vi>)  [unwired: 1 out]
        }
      }
      n5 = call <vilib>:"Has LLB Extension.vi"("path"=w20) -> ("path to VI library?"=w19:bool)
      n6 = Format Into String(format string="%s.lvclass", w15) -> (resulting string=w27:string)  [unwired: 2 in, 1 out]
      n7 = Search and Replace String(replace all?=TRUE ("replace all? (F)"), input string=w13, search string="EmptyClass", replace string=w15) -> (result string=w14:string)  [unwired: 4 in, 3 out]
      n8 = case shown="False" w19 {
        tunnel: [w42 w52] -> w26
        tunnel: w20 -> [w39 w51]
        tunnel: w27 -> [w43 w53]
        tunnel: [w41 w54] -> w25
        tunnel: w24 -> [w40 w49]
        tunnel: w15 -> [_ _]
        tunnel: w14 -> [w37 _]
        frame False {
          n9 = call <vilib>:"Create Directory Recursive.vi"("directory"=w39) -> ("directory copy"=w38:path)  [unwired: 4 in, 2 out]
          n10 = Build Path(base path=w38, name or relative path=w43) -> (appended path=w42:path)
          n11 = Write to Text File(file (use dialog)=w42, text=w37, error in=w40) -> (error out=w41:errorcluster)  [unwired: 1 in, 2 out]
        }
        frame True {
          w44 = "RSRC\r\n\u0000\u0003LVARLBVW\u0000\u0000=Ì\u0000\u0000\u0001ó\u0000\u0000\u0000 \u0000\u0000=¬\u0000\u0000\u0000\u0004\u0000\u0000\u0000\u0000\u0000\u0000\u0000\u0004\u0000\u0000\u0000\u0000\u0000\u0000\u0000\u0004\u0000\u0000\u0000\u0000\u0000\u0000\u0000\u0004\u0000\u0000\u0000\u0000\u0000\u0000\u0000\u0000\u0000\u0000\u0000\u0000\u0000\u0000\u0000\u0000\"\u0000\u0000\u0000>\u0000\u0000\u0003æ\u0000\u0000\u0018>\u0000\u0000\u0018\"\u0000\u0000\u0000\u0000\u0000\u0000\u001fÿÿø\u0000\u0000\u0000\u0000\u0000\u0000\u0000\u0000\u0000@\u0000\u0000\u0004\u0004\u0000\u0000\u0000à\u0001À\u0001\u0002 \u0002\u0005Ð\nJ\u0005Ð\u0002\b\u0005Ð\u0001\u0010\u0002 \u0000à\u0001À\u0000\u0000\u0000\u0000\u0007þ\u0001à\u0002B\u001a\u0010\u0006¢\u0002\u0010\u0003&\u001a\u0010\u0006*\u0003ð\u0002\u0012\u001bð\u0007þ\u0003ð\u0002ª\u001bð\u0000\u0000\u0001à\u0000\u0000\u0000\u0000\u0000\u0000\u0000\u0000\u0000\u0000\u0000\u0000\u0000\u0000\u0000\u0000\u0000\u0000\u0000\u0000\"\u0000\u0000\u0000>\u0000\u0000\u0003æ\u0000\u0000\u0018>\u0000\u0000\u0018\"\u0000\u0000\u0000\u0000\u0000\u0000\u001fÿÿø\u0000\u0000\u0000\u0000\u0000\u0000\u0000\u0000\u0006\u0000\u001fð\u0005\u0010\u0010\u0004`\u0012\u0004\u0014P\u0005Ä\u0011\u0010\u0004\u0014P\u0004`\u0012\u0005\u0010\u0010\u0006\u0000\u001fð\u0000\u0000\u0000\u0000\u0007ü\u0018\u0000\u0004\u0004\u0016\u0000\u0005\u0011\u0005\u0010`\u0006L\u0016\u0010\u0006L\u0010`\u00044\u0011\u00044\u0016\u0000\u0007ü\u0018\u0000\u0000\u0000\u0000\u0000\u0000\u0000\u0000\u0000\u0000\u0000\u0002\u0000\u0000\u0000\u0000\u0000\u0000\u0000\u0000\u0000\u0000\u0000\u0000\u0000\u0000\u0000\u0000\u0000\u0000\u0000\u0000\u0000\u0000\u0000\u0000\u0000\u0000\u0000\u0000\u0000\u0000\u0000\u0000\u0000\u0000\u0000\u0000\u0000\u0000ð\u0000ð\u0000\u0000\u0000\u0000\u0000\u0000\u0000\u0000\u0000\u0000\u0000\u0000\u0000ÿÿð\u0000\u0000\u0000\u0000\u0000\u0000\u0000\u0000\u0000\u0000\u0000ÿÿð\u000fð\u0000\u0000\u0000\u0000\u0000\u0000\u0000\u0000\u0000\u000fð\u0000\u0000ÿÿð\u0000\u0000\u0000\u0000\u0000\u0000\u0000\u0000\u0000\u000fð\u0000\u0000ð\u0000ð\u0000\u0000\u0000\u0000\u0000\u0000\u0000\u0000\u0000\u0000\u0000\u0000\u0000\u0000\u0000\u0000\u0000\u0000\u0000\u0000\u0000\u0000\u0000\u0000\u0000\u000fÿÿÿÿÿÿÿÿÿÿÿÿð\u0000\u0000\u0000\u0000\u0000\u0000\u0000\u0000\u0000\u0000\u0000\u0000\u0000\u0000\u0000\u0000\u0000\u0000\u0000\u0000\u0000\u0000\u0000\u0000\u0000\u0000\u0000\u0000\u0000\u0000\u0000\u0000\u0000\u0000\u0000\u0000\u0000\u000f\u0000\u0000\u0000\u0000\u0000\u0000\u0000\u0000\u0000\u0000\u0000\u0000\u0000\u000f\u0000\u0000\u0000\u000f\u0000\u0000\u0000\u0000\u0000\u0000\u0000\u0000\u0000\u0000\u0000\u0000\u0000ÿð\u0000\u0000\u0000\u0000\u0000\u000fÿ\u0000\u0000\u0000\u0000\u0000\u0000\u000f0Ï\u0000\u0000\u0000\u0000\u0000üÌð\u0000\u0000\u0000\u0000\u0000ð<Íð\u0000\u0000\u0000\u000fÈøß\u0000\u0000\u0000\u0000ððÃÍðð\u0000\u0000\u000fÏ..."  # EmptyClass.lvclass in LLB
          n12 = Strip Path(path=w51) -> (stripped path=w50:path)  [unwired: 1 out]
          n13 = call <vilib>:"Create Directory Recursive.vi"("error in (no error)"=w49, "directory"=w50) -> ("error out"=w48:errorcluster)  [unwired: 3 in, 2 out]
          n14 = Write to Text File(file (use dialog)=w51, text=w44, error in=w48) -> (error out=w46:errorcluster)  [unwired: 1 in, 2 out]
          n15 = Build Path(base path=w51, name or relative path="EmptyClass.lvclass") -> (appended path=w45:path)
          n16 = call <vilib>:"Librarian Rename.vi"("error in (no error)"=w46, "new name"=w53, "path"=w45) -> ("error out"=w54:errorcluster, "new path"=w52:path)  [unwired: 7 in]
        }
      }
      n17 = invoke class="ProjectItem" method="AddItem"(reference=w32, error in=w25, "Name"=w27, "Path"=w26, "Type"="LVClass") -> (reference out=w28:refnum<vi>, error out=w23:errorcluster, "AddItem"=w29:refnum<vi>)  [unwired: 1 in, 3 out]
      n18 = Unbundle(w23) -> ("status"=w18:bool)  [unwired: 2 out]
      n19 = Or(x=w19, y=w18) -> ()  [unwired: 1 out]
      n20 = case shown="True" w18 {
        tunnel: w29 -> [w59 w62]
        tunnel: [w55 w67] -> w12
        tunnel: w25 -> [w58 w60]
        tunnel: [w57 w64] -> w22
        tunnel: w30 -> [_ w69]
        tunnel: w26 -> [_ w61]
        frame False {
          w56 = refnum<vi> refnum  # LVClassLibrary
          n21 = To More Specific Class(target class=w56, reference=w59, error in=w58) -> (specific class reference=w55:refnum<vi>, error out=w57:errorcluster)
        }
        frame True {
          # "Is it a Autopopulating folder?"
          n22 = Close Reference(reference=w62, error in (no error)=w60) -> ()  [unwired: 1 out]
          n23 = property class="Project"(reference=w69, error in=w60) -> (error out=w66:errorcluster, "App Ref"=w68:refnum<vi>)  [unwired: 1 out]
          n24 = invoke class="App" method="LVClass.Open"(reference=w68, error in=w66, "Path"=w61) -> (reference out=w63:refnum<vi>, error out=w65:errorcluster, "LVClass.Open"=w67:refnum<vi>)  [unwired: 1 in, 1 out]
          n25 = Close Reference(reference=w63, error in (no error)=w65) -> (error out=w64:errorcluster)
        }
      }
      n26 = case shown="True" w33 {
        tunnel: w22 -> [w70 w73]
        tunnel: [w70 w72] -> w21
        tunnel: w28 -> [_ w71]
        frame False {
        }
        frame True {
          n27 = Close Reference(reference=w71, error in (no error)=w73) -> (error out=w72:errorcluster)
        }
      }
    }
    frame Error {
    }
  }
  "Project Refnum Out" <- w6
  "error out" <- w10
  "Class Refnum Out" <- w2
  "ClassPathOut" <- w3
